vi "Language Editor.vi"(8 "error in (no error)":errorcluster, 11 "Top Level VI":refnum<vi>) -> (0 "error out":errorcluster)   [LabVIEW 2019, in "Language Editor.lvlib"]
doc: "- - -\nCopyright (c) 2026, Merecs Engineering GmbH"
uses:
  Language Editor.lvlib
  type defs/Enum Class Name.ctl
  Language Selection/TypeDefs/Cluster Language Configuration.ctl
  Language Selection/community/Cluster Settings Data.ctl
  Language Selection/TypeDefs/Cluster Language.ctl
  Language Selection/TypeDefs/Cluster PropertyTranslation.ctl
  Language Selection/TypeDefs/Enum Property Type.ctl
  type defs/Cluster VI controls.ctl
  type defs/Cluster Translations.ctl
  <vilib>/Utility/miscctls.llb/LVPointTypeDef.ctl
  <vilib>/Utility/miscctls.llb/LVRowAndColumnUnsignedTypeDef.ctl
  <vilib>/Utility/miscctls.llb/LVBoundsTypeDef.ctl
  <vilib>/Utility/miscctls.llb/LVMapReplaceAction.ctl
  70223300-0df1-46fa-af21-f54e94af5b86.vi
  <vilib>/addons/Tools/Unicode/_subVIs/Convert UTF-16LE to ASCII (Scalar).vi
  Language Selection/Language Selection.lvlib
  <vilib>/addons/Tools/Unicode/UI Unicode Tools.lvlib
  <vilib>/Utility/LVLibp/NI_PackedLibraryUtility.lvlib
panel:
  in  "Import":bool
  in  "Export to txt":bool
  in  "App File Path":path=path "C:/Projects/Base/Modules/Language Toolkit" caption="Application Base Folder Path"
  in  "Save As":bool
  in  "Language Config Path":path=path "C:/Projects/Base/Modules/Language Toolkit/data/Language Translation_default.json"
  in  "Save Settings":bool
  in  "Init":bool
  in  "Exit":bool
  in  "Tab Control":T1(tab)
  in  "StartLang":string(combo) caption="Startup Language"
  in  "DefLang":string(combo) caption="Default Language"
  in  "Delete":bool
  in  "AddLanguage":bool
  in  "Languages":i32(listbox) caption="Languages to translate"
  in  "Search":string
  in  "AllLanguages":i32(listbox)=-1 caption="List of languages"
  in  "VI.DelAllFilter":bool
  in  "Button.GoToTranslation":bool
  in  "Add VI":bool caption="Last"
  in  "Sort VIs":bool
  in  "Delete VI":bool caption="First"
  in  "Button.AddToFPTranslation":bool
  in  "ControlsFilter":T2={"VI.Filter.Label"="num", "VI.Filter.Class"="", "No Error Cluster"=TRUE, "NonTranslated"=TRUE, "OnlyVisibleArea"=TRUE} caption="Controls Filter"
  in  "Controls":i32[](listbox)
  in  "VIs":i32(listbox) caption="VIs to translate"
  out "IsCtrlVisible":bool
  in  "Search Label":string
  in  "DelFilter":bool
  out "Warning":string
  in  "FPT.TextUnicode":string caption="Translation"
  in  "CTRL Index":i32 caption="Control Index" min=0 max=26 step=1
  in  "ListOfControls":i32(listbox) caption="List Of Controls"
  out "Caption Unvisible":bool
  in  "FP Translation Comment":string caption="Comment"
  out "IsCtrlUsed":bool
  out "Class Name":T3=enum."ListBox"
  in  "Button.NextUnusedCtrls":bool
  in  "VIs with Ctrl":i32(listbox) caption="List of UIs with control:"
  in  "Button.ZoomToCtrl":bool
  out "2D Picture":picture
  in  "Tree":string(tree)="TipStrip"
  in  "DelCtrlToTranslate":bool caption="First"
  in  "AddCtrlToTranslate":bool caption="Last"
  in  "Label":string="L.Listbox"
  in  "FPT.TextANSI":string caption="Translation"
  out "IsCtrlInUIArea":bool
  in  "TT.TextUnicode":string caption="Translation"
  in  "TextTranslation":i32(listbox)
  in  "TT.TextANSI":string caption="Translation"
  in  "ListOfTextTranslations":i32(listbox)=-1
  in  "DeleteText":bool caption="First"
  in  "AddTextToTranslate":bool caption="Last"
  in  "TextName":string="L.Listbox" caption="Name"
  in  "Search text":string
  # "Select Language"
  # "Language Preferences"
  # "Double Click to Show VI Frontpanel"
  # "Connector Pane"
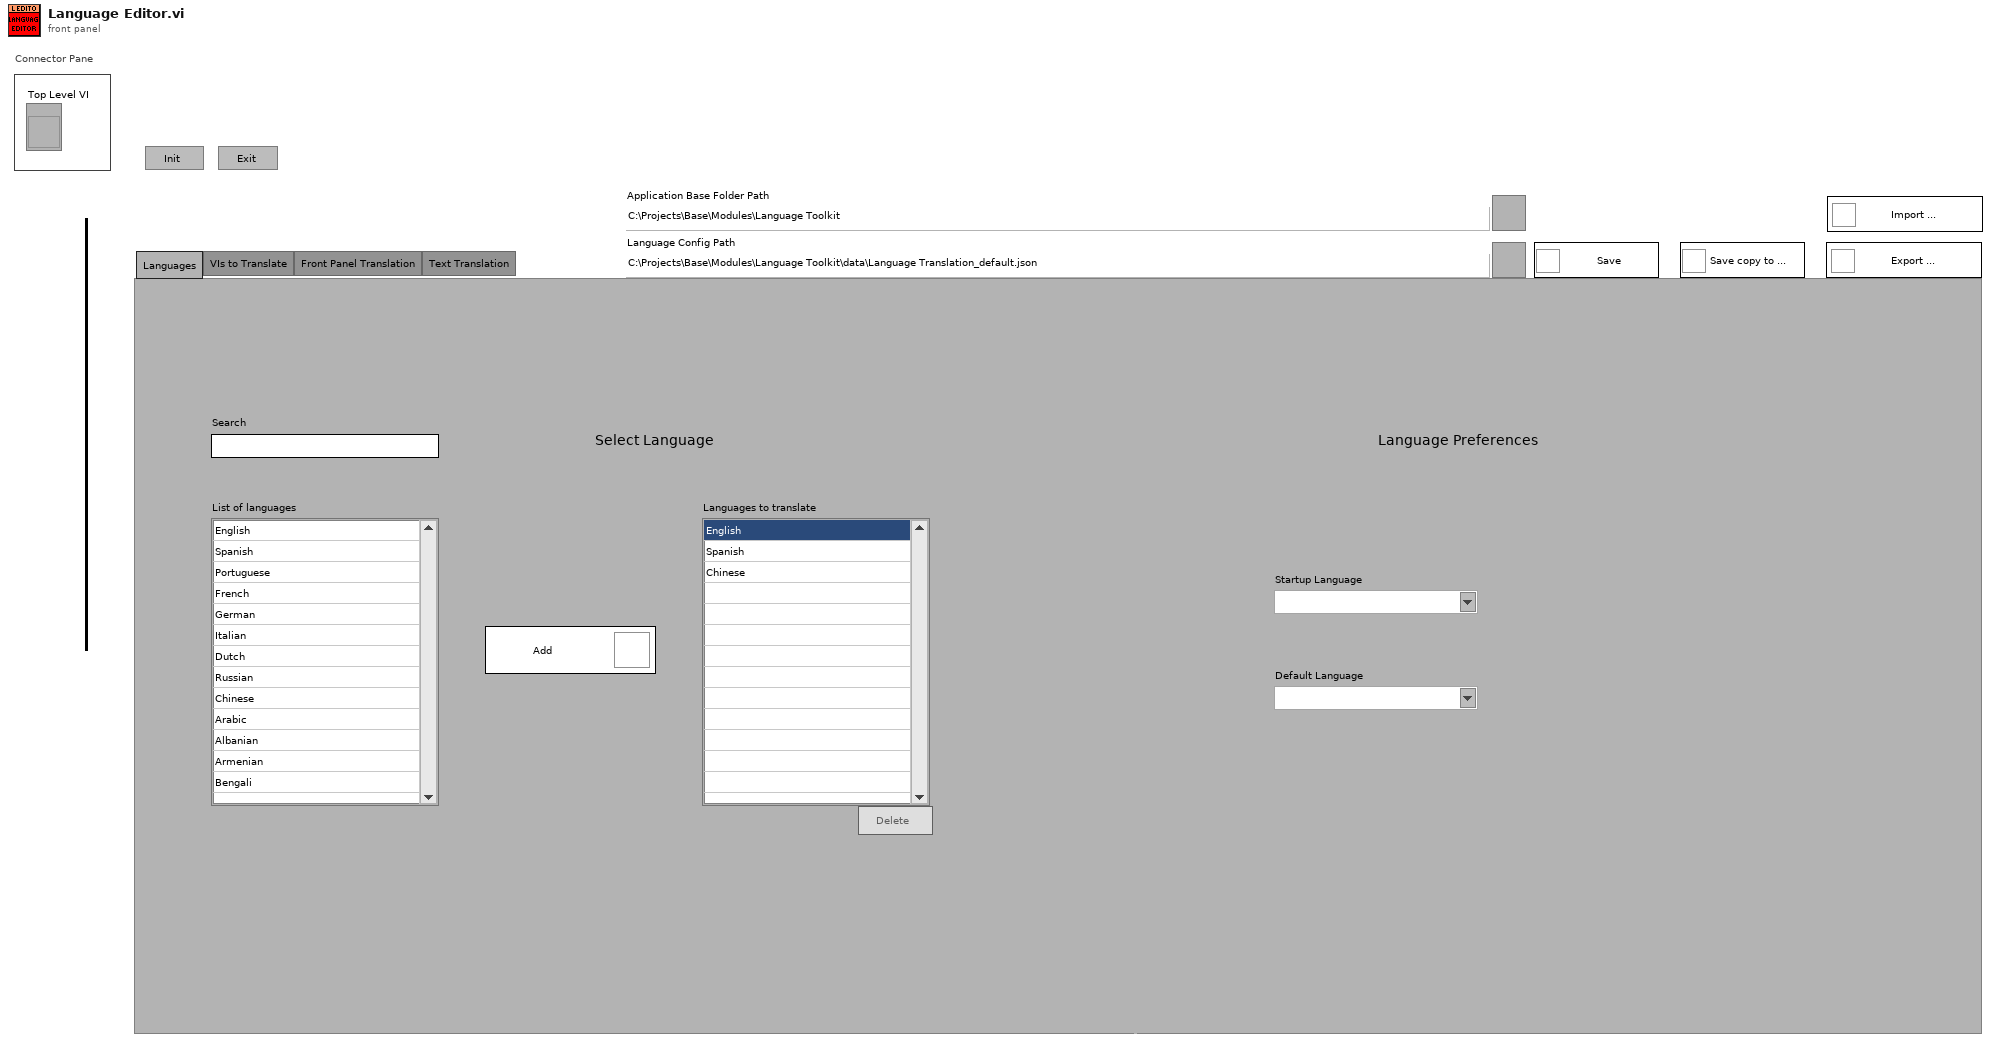
[diagram p1: front panel]
types:
  T1 = enum32{"Languages", "VIs to Translate", "Front Panel Translation", "Text Translation"}
  T2 = cluster{"VI.Filter.Label":string, "VI.Filter.Class":string, "No Error Cluster":bool, "NonTranslated":bool, "OnlyVisibleArea":bool}
  T3 = typedef "Language Editor.lvlib/Enum Class Name.ctl" = enum16{"Default Control", "Boolean", "ListBox", "Table", "Graph", "Array", "Ring", "String", "TabControl", "ComboBox", "TreeControl"}
  T4 = enum8{"Enabled", "Disabled", "Disabled and Grayed Out"}
  T5 = enum32{"Invalid", "Standard", "Closed", "Hidden", "Minimized", "Maximized"}
  T6 = enum32{"invalid app kind", "Development System", "Run Time System", "Student Edition", "Embedded LabVIEW", "Evaluation", "Custom"}
  T7 = typedef "Language Selection.lvlib/Cluster Language.ctl" = cluster{"Label":string, "Comment":string, "Property":T8[]}
  T8 = typedef "Language Selection.lvlib/Cluster PropertyTranslation.ctl" = cluster{"Type":T9, "Translation ANSI":string[], "Translation Unicode":string[]}
  T9 = typedef "Language Selection.lvlib/Enum Property Type.ctl" = enum16{"NA", "Caption", "String Value", "Boolean Text", "Ring Strings", "1D Array Elements", "2D Array Elements", "(MC)Listbox Header", "(MC)Listbox Items", "Tab Pages Names", "X & Y GraphChart", "Plot Names", "Table Headers", "Table Items", "TipStrip", "Combobox Strings", "Cursor Name", "Tree Col Headers"}
  T10 = typedef "LVPointTypeDef.ctl" = cluster{"Horizontal":i16, "Vertical":i16}
  T11 = typedef "LVRowAndColumnUnsignedTypeDef.ctl" = cluster{"Row":u32, "Column":u32}
  T12 = typedef "LVBoundsTypeDef.ctl" = cluster{"Width":u32, "Height":u32}
  T13 = typedef "LVMapReplaceAction.ctl" = enum32{"Modify Entry only if found", "Add or Modify Entry", "Delete Entry"}
  T14 = typedef "Language Editor.lvlib/Cluster Translations.ctl" = cluster{"Tags":string, "Comment":string, "Properties":T8[]}
  T15 = typedef "Language Selection.lvlib/Cluster Language Configuration.ctl" = cluster{"Data":T16, "Supported Languages":cluster{"ANSI":string[], "Unicode":string[]}, "VIs":path[], "FP Translations":T7[], "Text Translations":T7[]}
  T16 = typedef "Language Selection.lvlib/Cluster Settings Data.ctl" = cluster{"Startup Language":string, "Default Language":string, "Languages":cluster{"ANSI":string[], "Unicode":string[]}}
  T17 = typedef "Language Editor.lvlib/Cluster VI controls.ctl" = cluster{"Label":string, "Class Name":string, "Type":string, "Tags":string, "refVI":refnum<vi>, "refCtl":refnum<vi>, "PageOfTab":string, "refPane":refnum<vi>}
  T18 = cluster{"Core":cluster{"Current VI Reference":refnum<vi>, "Close Panel on Exit?":bool}, "LT":T15, "CTRLs":map{path, T17[]}, "Controls":cluster{"Item Names":string[][], "Item Symbols":i32[]}, "Selected CTRLs":T17[], "OldVal.ListOfVIs":string, "ZoomOutFactor":dbl, "FP.Tr":map{string, T14}, "T.Tr":map{string, T14}, "Origin":T10}
  T19 = cluster{"Current VI Reference":refnum<vi>, "Close Panel on Exit?":bool}
  T20 = cluster{"Item Names":string[][], "Item Symbols":i32[]}
  T21 = cluster{"Left Cell String":string, "Child Text":string[], "Child Tag":string, "Item Indent":i32, "Child Only?":bool, "Glyph Index":i32}[]
  T22 = cluster{"left":i16, "top":i16, "right":i16, "bottom":i16}
  T23 = enum16{"open", "replace", "create", "open or create", "replace or create", "replace or create with confirmation"}
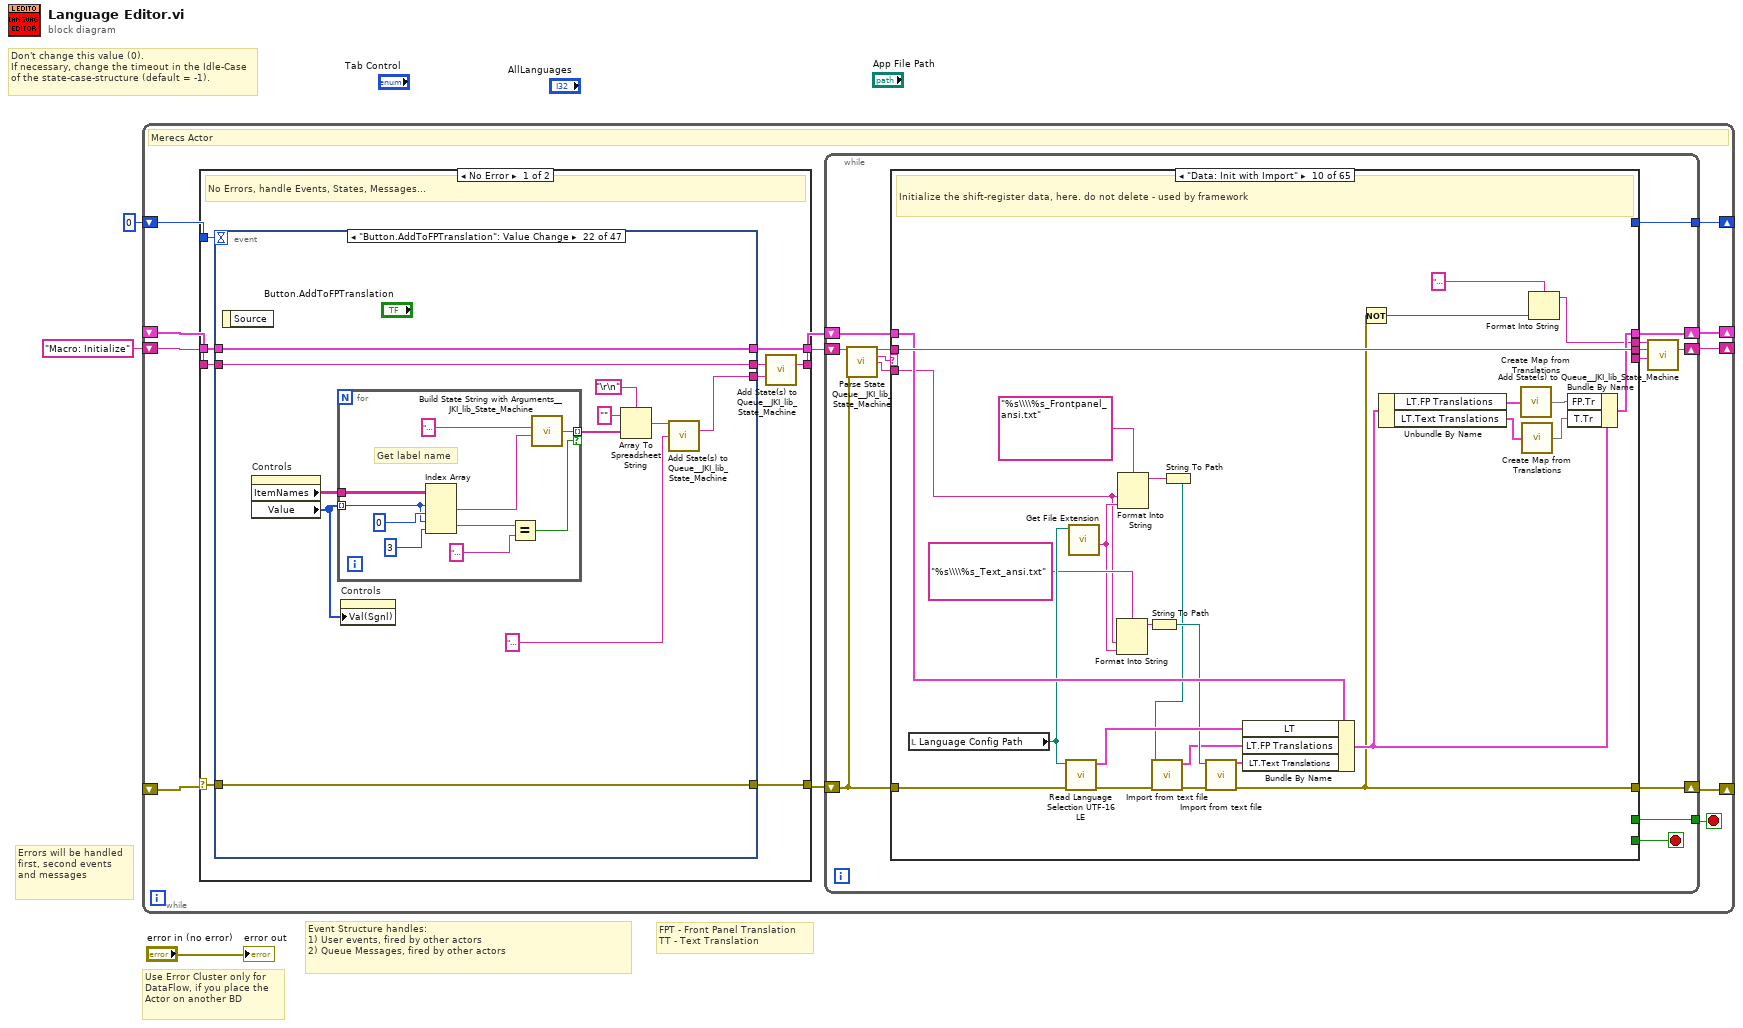
[diagram p0: block diagram]
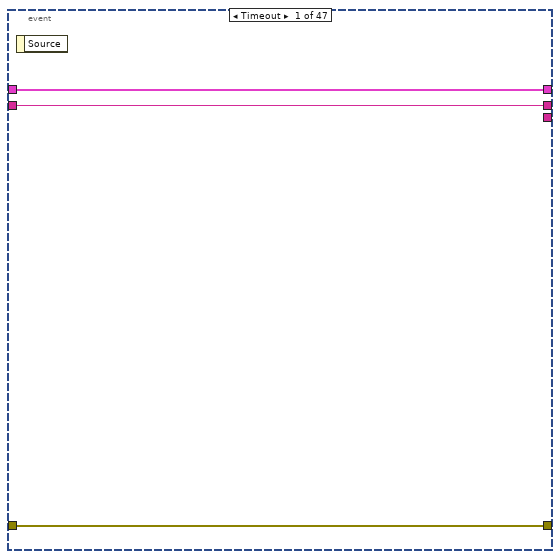
[diagram p2: hidden frame]
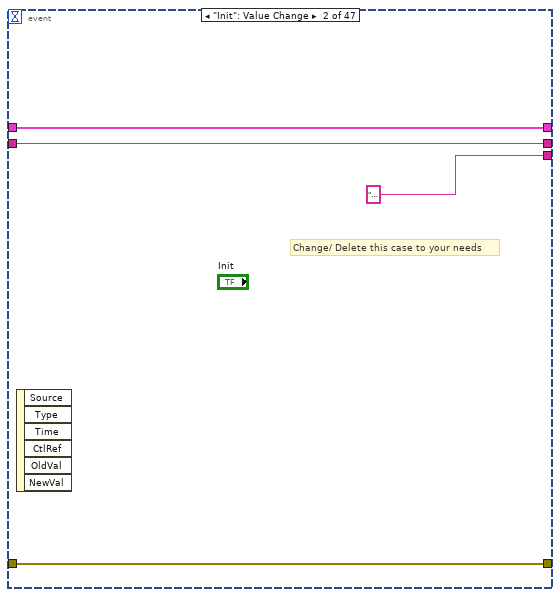
[diagram p3: hidden frame]
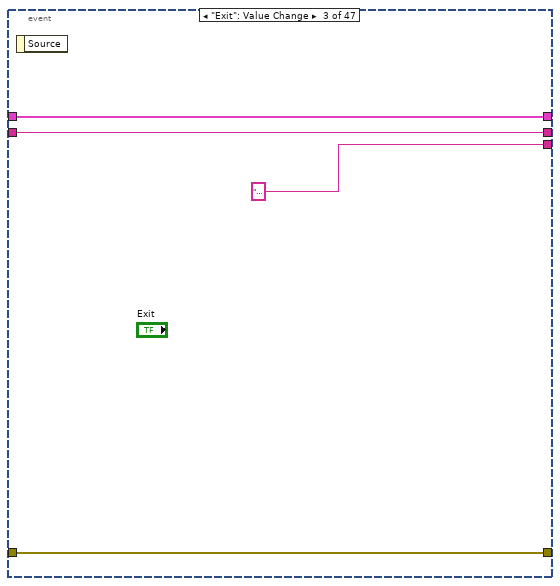
[diagram p4: hidden frame]
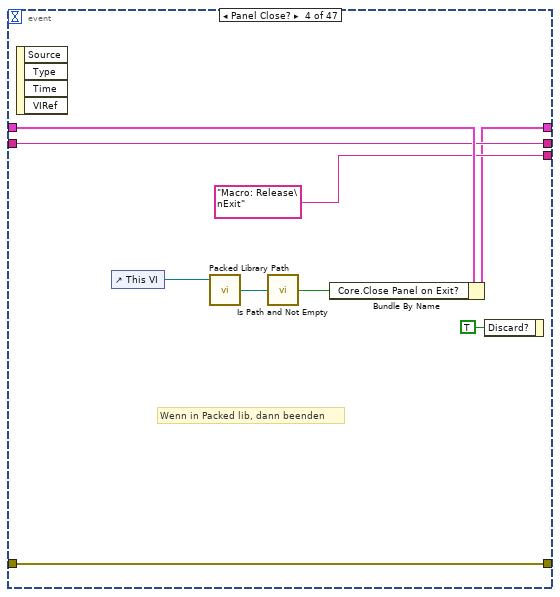
[diagram p5: hidden frame]
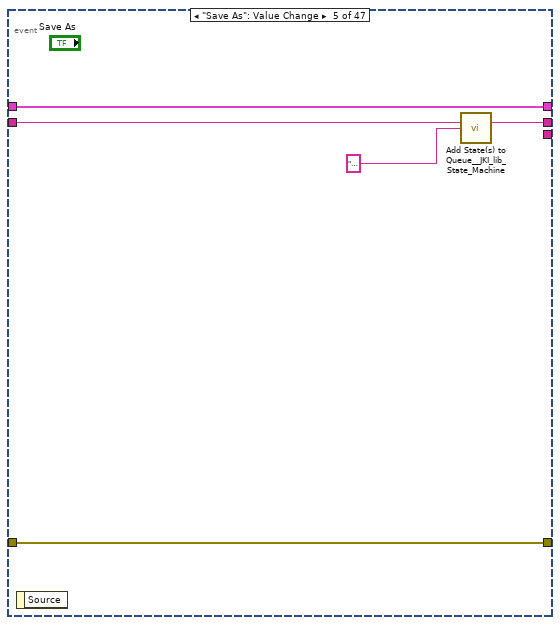
[diagram p6: hidden frame]
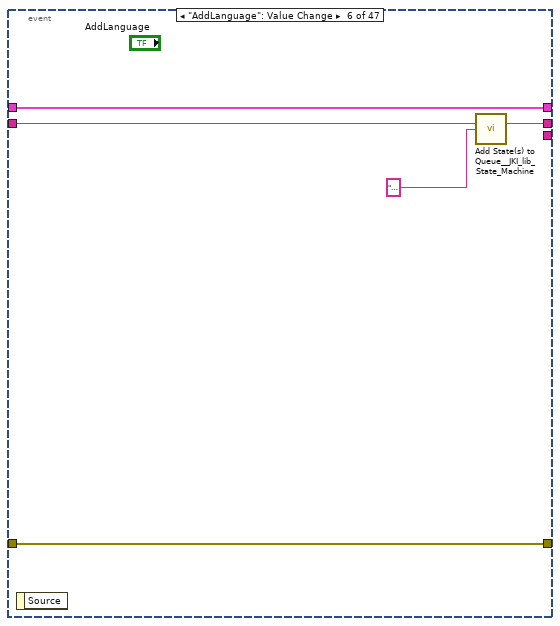
[diagram p7: hidden frame]
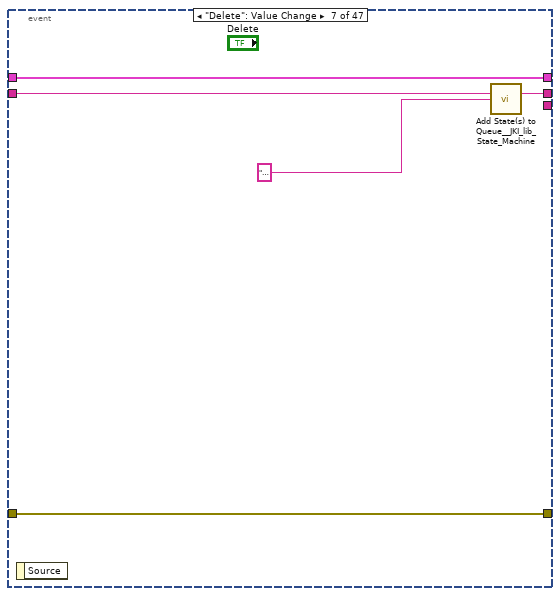
[diagram p8: hidden frame]
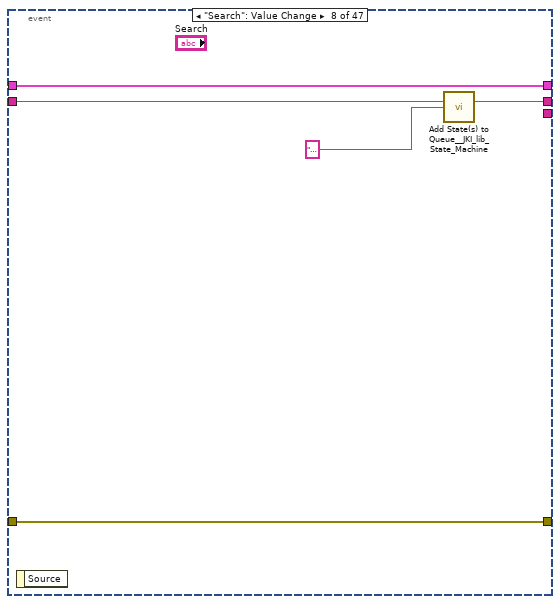
[diagram p9: hidden frame]
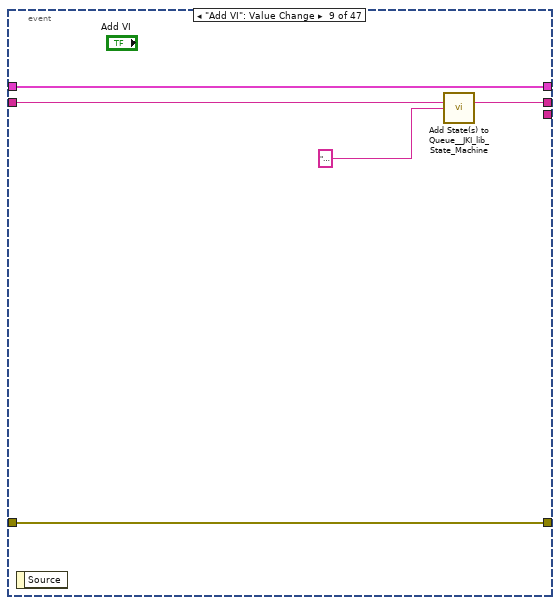
[diagram p10: hidden frame]
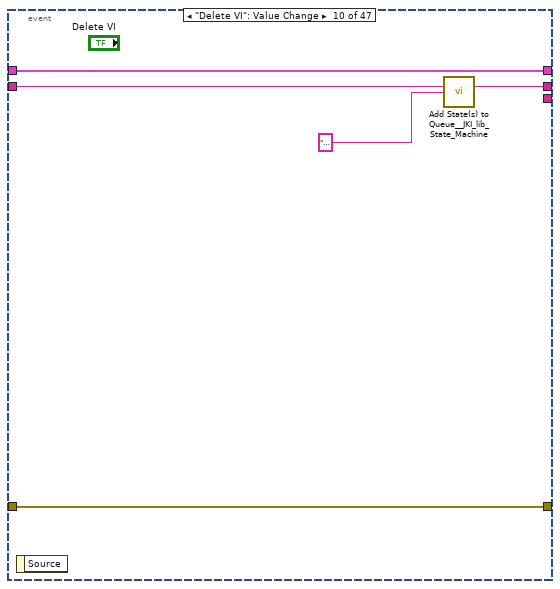
[diagram p11: hidden frame]
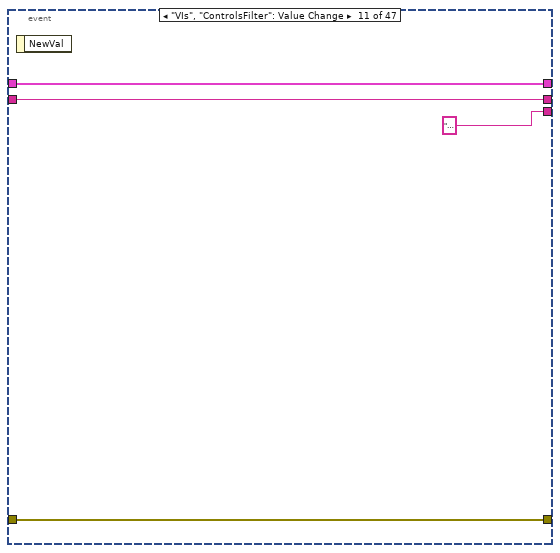
[diagram p12: hidden frame]
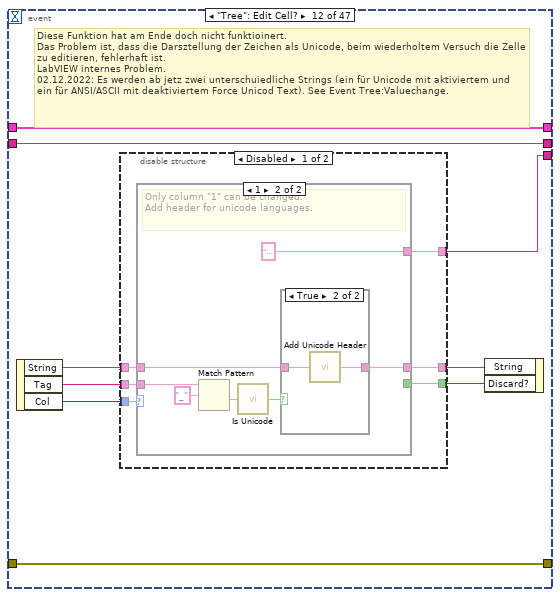
[diagram p13: hidden frame]
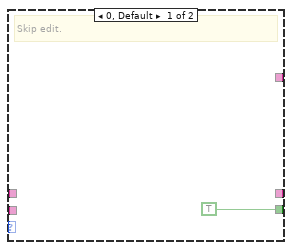
[diagram p14: hidden frame]
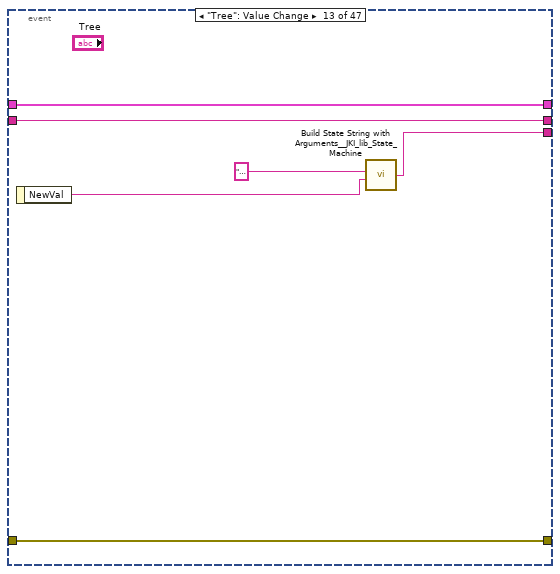
[diagram p17: hidden frame]
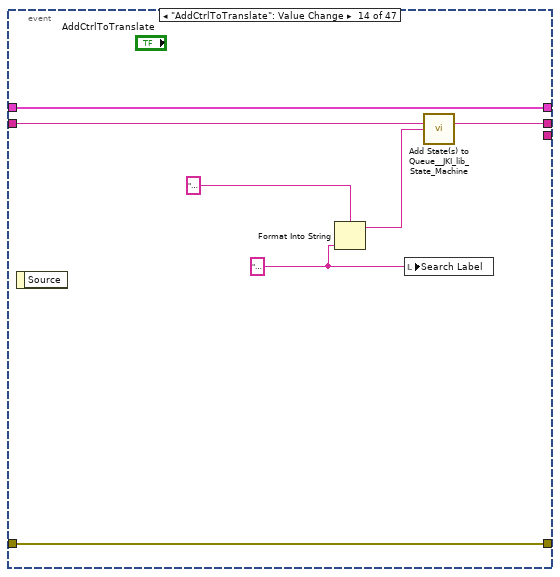
[diagram p18: hidden frame]
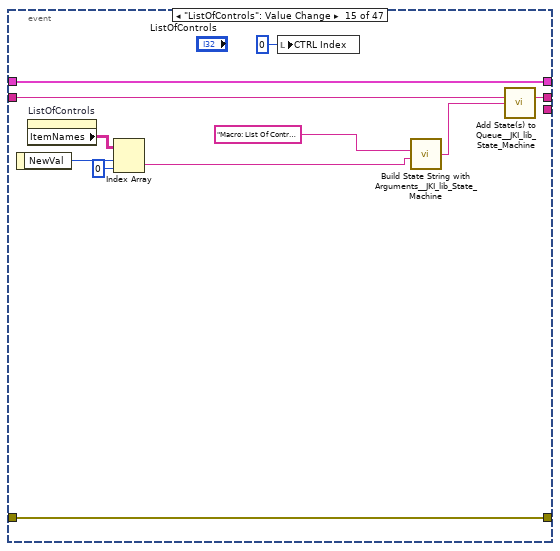
[diagram p19: hidden frame]
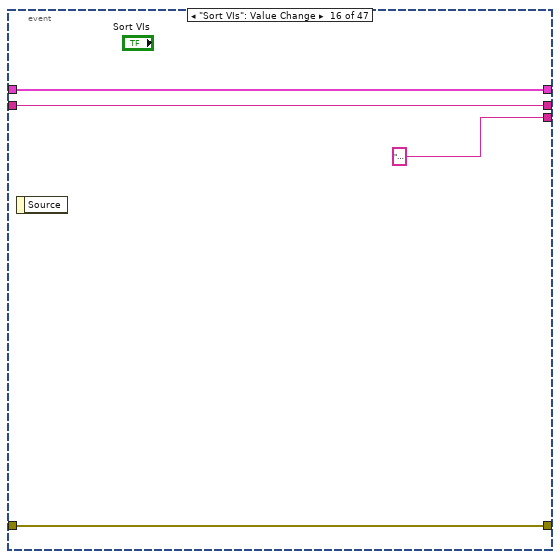
[diagram p20: hidden frame]
diagram:
  # "FPT - Front Panel Translation\nTT - Text Translation"
  # "Errors will be handled first, second events and messages"
  # "Use Error Cluster only for DataFlow, if you place the Actor on another BD"
  # "Event Structure handles:\n1) User events, fired by other actors\n2) Queue Messages, fired by other actors"
  # "Don't change this value (0).\nIf necessary, change the timeout in the Idle-Case of the state-case-structure (default = -1)."
  n1 = while {
    shift-right: [w15] -> _
    shift-left: _ -> [w13]
    shift-right: [w5] -> _
    shift-left: 0 -> [w8]
    shift-right: [w7] -> _
    shift-left: "Macro: Initialize" ("States Out") -> [w6]
    shift-right: [w14] -> _
    shift-left: _ -> [w4]
    stop <- w10 stop-if-true
    # "Merecs Actor"
    n2 = case shown="No Error" w4 {
      selector: w4 -> [w19 w362]
      tunnel: w13 -> [w24 w364]
      tunnel: [w23 w364] -> w12
      tunnel: [w18 w363] -> w11
      tunnel: [w22 w362] -> w9
      tunnel: w8 -> [w21 _]
      tunnel: w6 -> [w20 w363]
      frame No Error {
        # "No Errors, handle Events, States, Messages..."
        n3 = event shown="[21] \"Button.AddToFPTranslation\": Value Change" {
          selector: _ -> [_ _ _ _ _ _ _ _ _ _ _ _ _ _ _ _ _ _ _ _ _ _ _ _ _ _ _ _ _ _ _ _ _ _ _ _ _ _ _ _ _ _ _ _ _ _ _]
          dyn-events: _ -> [_ _ _ _ _ _ _ _ _ _ _ _ _ _ _ _ _ _ _ _ _ _ _ _ _ _ _ _ _ _ _ _ _ _ _ _ _ _ _ _ _ _ _ _ _ _ _]
          timeout: w21 -> [_ _ _ _ _ _ _ _ _ _ _ _ _ _ _ _ _ _ _ _ _ _ _ _ _ _ _ _ _ _ _ _ _ _ _ _ _ _ _ _ _ _ _ _ _ _ _]
          tunnel: w24 -> [w27 w31 w34 w43 w49 w54 w59 w64 w69 w74 w78 w87 w110 w117 w128 w132 w140 w145 w150 w155 w162 w173 w189 w197 w201 w205 w214 w221 w230 w234 w238 w242 w246 w250 w254 w266 w276 w283 w287 w294 w324 w328 w332 w336 w344 w349 w357]
          tunnel: [w27 w31 w34 w37 w49 w54 w59 w64 w69 w74 w78 w87 w110 w117 w128 w132 w140 w142 w147 w155 w162 w173 w189 w197 w201 w205 w209 w221 w230 w234 w238 w242 w246 w250 w254 w266 w276 w283 w287 w294 w324 w328 w332 w336 w344 w349 w357] -> w23
          tunnel: [w25 w28 w32 w41 w46 w50 w56 w62 w67 w72 w77 w86 w109 w115 w125 w131 w139 w144 w149 w154 w161 w172 w188 w196 w200 w204 w211 w220 w229 w233 w237 w241 w245 w249 w253 w265 w275 w282 w286 w293 w323 w327 w331 w335 w343 w348 w356] -> w16
          tunnel: w19 -> [w26 w30 w35 w44 w48 w53 w58 w63 w68 w73 w76 w85 w108 w116 w127 w130 w138 w143 w148 w153 w160 w171 w187 w195 w199 w203 w213 w219 w228 w232 w236 w240 w244 w248 w252 w264 w274 w281 w285 w292 w322 w326 w330 w334 w342 w347 w351]
          tunnel: [w26 w30 w35 w44 w48 w53 w58 w63 w68 w73 w76 w85 w108 w116 w127 w130 w138 w143 w148 w153 w160 w171 w187 w195 w199 w203 w213 w219 w228 w232 w236 w240 w244 w248 w252 w264 w274 w281 w285 w292 w322 w326 w330 w334 w342 w347 w350] -> w22
          tunnel: w20 -> [w25 w28 w32 w41 w47 w51 w57 w61 w66 w71 w77 w86 w109 w114 w126 w131 w139 w144 w149 w154 w161 w172 w188 w196 w200 w204 w210 w220 w229 w233 w237 w241 w245 w249 w253 w265 w275 w282 w286 w293 w323 w327 w331 w335 w343 w348 w356]
          tunnel: [_ "Macro: Initialize" ("State(s) at Back (\"\")") "Macro: Release\nExit" ("State(s) at Back (\"\")") "Macro: Release\nExit" ("State(s) at Back (\"\")") _ _ _ _ _ _ "UI: VIs Update Controls" ("State") w79 w105 _ _ "VIs: Sort\nUI: VIs Update" ("State with Arguments") w134 _ _ _ "UI: VIs Update Controls" ("State with Arguments") w169 "FP Translation: Edit Properties\nUI: FP Translation Filter ListOfControls" ("State with Arguments") "FP Translation: Edit Properties\nUI: FP Translation Filter ListOfControls" ("State with Arguments") "FP Translation: Delete Control" ("State") "FP Translation: Look for Next unused CTRL" _ w216 w222 "Data: FP Translation Edit Comment" ("State") "UI: FP Translation Filter ListOfControls" ("State") "Text Translation: Show Translation\nText Translation: Value Change" ("State") "Text Translation: Add Text >> New Text" ("State(s) at Back (\"\")") "Text Translation: Delete Text" ("State(s) at Back (\"\")") "Text Translation: Value Change" ("f") "Text Translation: Edit Properties" ("State(s) at Back (\"\")") "Text Translation: Edit Properties" ("State(s) at Back (\"\")") w278 "Data: Update Config\nData: Save" ("State with Arguments") _ w314 "VIs: Show Frontpanel" ("State with Arguments") "Text Translation: Filter" ("State with Arguments") _ w338 "General: Export to txt" ("f") w355] -> w17
          event Timeout {
            n4 = event-data() -> ()  [unwired: 1 in, 1 out]
          }
          event "Init": Value Change {
            # "Change/ Delete this case to your needs"
            n5 = event-data() -> ()  [unwired: 1 in, 6 out]
          }
          event "Exit": Value Change {
            n6 = event-data() -> ()  [unwired: 1 in, 1 out]
          }
          event Panel Close? {
            # "Wenn in Packed lib, dann beenden"
            n7 = event-data() -> ()  [unwired: 1 in, 4 out]
            n8 = control-ref of="This VI"() -> (w39:refnum<vi>)
            n9 = call <vilib>:"Packed Library Path.vi"("vi reference"=w39) -> ("packed library path"=w38:path)  [unwired: 2 in, 2 out]
            n10 = call <vilib>:"Is Path and Not Empty.vi"("path"=w38) -> ("Is Path and Not Empty?"=w36:bool)  [unwired: 4 in]
            n11 = Bundle By Name(cluster=w43, "Core.Close Panel on Exit?"=w36) -> (w37:T18)
            n12 = event-data("Discard?"=TRUE) -> ()  [unwired: 1 in, 1 out]
          }
          event "Save As": Value Change {
            n13 = event-data() -> ()  [unwired: 1 in, 1 out]
            n14 = call <vilib>:"Add State(s) to Queue__JKI_lib_State_Machine.vi"("State(s) in (\"\")"=w47, "State(s) at Back (\"\")"="General: File Save As" ("State(s) at Back (\"\")")) -> ("States Out"=w46:string)  [unwired: 13 in]
          }
          event "AddLanguage": Value Change {
            n15 = event-data() -> ()  [unwired: 1 in, 1 out]
            n16 = call <vilib>:"Add State(s) to Queue__JKI_lib_State_Machine.vi"("State(s) in (\"\")"=w51, "State(s) at Back (\"\")"="Languages: Add\nUI: Languages" ("State(s) at Back (\"\")")) -> ("States Out"=w50:string)  [unwired: 13 in]
          }
          event "Delete": Value Change {
            n17 = event-data() -> ()  [unwired: 1 in, 1 out]
            n18 = call <vilib>:"Add State(s) to Queue__JKI_lib_State_Machine.vi"("State(s) in (\"\")"=w57, "State(s) at Back (\"\")"="Languages: Delete\nUI: Languages" ("State(s) at Back (\"\")")) -> ("States Out"=w56:string)  [unwired: 13 in]
          }
          event "Search": Value Change {
            n19 = event-data() -> ()  [unwired: 1 in, 1 out]
            n20 = call <vilib>:"Add State(s) to Queue__JKI_lib_State_Machine.vi"("State(s) in (\"\")"=w61, "State(s) at Back (\"\")"="Languages: Search" ("State(s) at Back (\"\")")) -> ("States Out"=w62:string)  [unwired: 13 in]
          }
          event "Add VI": Value Change {
            n21 = event-data() -> ()  [unwired: 1 in, 1 out]
            n22 = call <vilib>:"Add State(s) to Queue__JKI_lib_State_Machine.vi"("State(s) in (\"\")"=w66, "State(s) at Back (\"\")"=" VIs: Add VI\nUI: VIs Update" ("State(s) at Back (\"\")")) -> ("States Out"=w67:string)  [unwired: 13 in]
          }
          event "Delete VI": Value Change {
            n23 = event-data() -> ()  [unwired: 1 in, 1 out]
            n24 = call <vilib>:"Add State(s) to Queue__JKI_lib_State_Machine.vi"("State(s) in (\"\")"=w71, "State(s) at Back (\"\")"="VIs: Delete VI\nUI: VIs Update" ("State(s) at Back (\"\")")) -> ("States Out"=w72:string)  [unwired: 13 in]
          }
          event "VIs", "ControlsFilter": Value Change {
            n25 = event-data() -> ()  [unwired: 1 in, 1 out]
          }
          event "Tree": Edit Cell? {
            # "Diese Funktion hat am Ende doch nicht funktioinert.\nDas Problem ist, dass die Darsztellung der Zeichen als Unicode, beim wiederholtem Versuch die Zelle zu editieren, fehlerhaft ist.\nLabVIEW internes Problem.\n02.12.2022: Es werden ab jetz zwei unterschuiedliche Strings (ein für Unicode mit aktiviertem und ein für ANSI/ASCII mit deaktiviertem Force Unicod Text). See Event Tree:Valuechange."
            n26 = event-data() -> ("String"=w81:string, "Tag"=w82:string, "Col"=w84:i32)  [unwired: 1 in]
            n27 = disable-structure shown="Disabled" {
              disable-tunnel: w84 -> [w93 _]
              disable-tunnel: [w92 _] -> w83
              disable-tunnel: w82 -> [w91 _]
              disable-tunnel: w81 -> [w90 _]
              disable-tunnel: [w89 _] -> w80
              disable-tunnel: [w88 _] -> w79
              frame Disabled {
                n28 = case shown="1" w93 {
                  tunnel: [TRUE _] -> w92
                  tunnel: w91 -> [_ w98]
                  tunnel: w90 -> [_ w97]
                  tunnel: [_ w96] -> w89
                  tunnel: [_ "FP Translation: Edit Properties" ("State with Arguments")] -> w88
                  frame 0, Default {
                    # "Skip edit."
                  }
                  frame 1 {
                    # "Only column \"1\" can be changed.\nAdd header for unicode languages."
                    n29 = Match Pattern(string=w98, regular expression="_") -> (after substring=w100:string)  [unwired: 1 in, 3 out]
                    n30 = call "Is Unicode.vi"("Language"=w100) -> ("Is Unicode"=w99:bool)
                    n31 = case shown="True" w99 {
                      tunnel: [w102 w103] -> w96
                      tunnel: w97 -> [w102 w104]
                      frame False {
                      }
                      frame True {
                        n32 = call "Add Unicode Header.vi"("Text"=w104) -> ("Text with header"=w103:string)
                      }
                    }
                  }
                }
              }
              frame Enabled {
              }
            }
            n33 = event-data("String"=w80, "Discard?"=w83) -> ()  [unwired: 1 in, 1 out]
          }
          event "Tree": Value Change {
            n34 = event-data() -> ("NewVal"=w106:string)  [unwired: 1 in]
            n35 = call <vilib>:"Build State String with Arguments__JKI_lib_State_Machine.vi"("Arguments (\"\")"=w106, "State"="UI: FP Translation Update Text Translations") -> ("State with Arguments"=w105:string)  [unwired: 4 in]
          }
          event "AddCtrlToTranslate": Value Change {
            w113 = "New Label" ("Search Label")
            n36 = event-data() -> ()  [unwired: 1 in, 1 out]
            n37 = Format Into String(format string="FP Translation: Add Control >> %s\nUI: FP Translation Filter ListOfControls" ("State(s) at Back (\"\")"), w113) -> (resulting string=w111:string)  [unwired: 2 in, 1 out]
            n38 = local write "Search Label"(w113) -> ()
            n39 = call <vilib>:"Add State(s) to Queue__JKI_lib_State_Machine.vi"("State(s) in (\"\")"=w114, "State(s) at Back (\"\")"=w111) -> ("States Out"=w115:string)  [unwired: 13 in]
          }
          event "ListOfControls": Value Change {
            n40 = event-data() -> ("NewVal"=w123:i32)  [unwired: 1 in]
            n41 = property on="ListOfControls" class="MCListbox (strict)"() -> ("ItemNames"=w121:string[][])  [unwired: 2 in, 2 out]
            n42 = Index Array(array=w121, index (row)=w123, index (col)=0 ("disabled index (col)")) -> (element=w119:string)
            n43 = local write "CTRL Index"(0 ("CTRL Index")) -> ()
            n44 = call <vilib>:"Build State String with Arguments__JKI_lib_State_Machine.vi"("Arguments (\"\")"=w119, "State"="Macro: List Of Controls Value Change") -> ("State with Arguments"=w120:string)  [unwired: 4 in]
            n45 = call <vilib>:"Add State(s) to Queue__JKI_lib_State_Machine.vi"("State(s) in (\"\")"=w126, "State(s) at Back (\"\")"=w120) -> ("States Out"=w125:string)  [unwired: 13 in]
          }
          event "Sort VIs": Value Change {
            n46 = event-data() -> ()  [unwired: 1 in, 1 out]
          }
          event "Label": Value Change {
            n47 = event-data() -> ("NewVal"=w133:string)  [unwired: 1 in]
            n48 = local write "Search Label"(w133) -> ()
            n49 = call <vilib>:"Build State String with Arguments__JKI_lib_State_Machine.vi"("Arguments (\"\")"=w133, "State"="FP Translation: Rename Control") -> ("State with Arguments"=w135:string)  [unwired: 4 in]
            n50 = call <vilib>:"Add State(s) to Queue__JKI_lib_State_Machine.vi"("State(s) in Front (\"\")"=w135, "State(s) in (\"\")"="UI: FP Translation Filter ListOfControls" ("State(s) in (\"\")")) -> ("States Out"=w134:string)  [unwired: 13 in]
          }
          event "StartLang": Value Change {
            n51 = event-data() -> ("NewVal"=w141:string)  [unwired: 1 in]
            n52 = Bundle By Name(cluster=w145, "LT.Data.Startup Language"=w141) -> (w142:T18)
          }
          event "DefLang": Value Change {
            n53 = event-data() -> ("NewVal"=w146:string)  [unwired: 1 in]
            n54 = Bundle By Name(cluster=w150, "LT.Data.Default Language"=w146) -> (w147:T18)
          }
          event "Languages": Value Change {
            n55 = event-data() -> ("NewVal"=w152:i32)  [unwired: 1 in]
            n56 = case shown="-1" w152 {
              tunnel: [T4."Disabled and Grayed Out" ("Disabled") T4."Enabled" ("Disabled")] -> w151
              frame -1 {
              }
              frame Default {
              }
            }
            n57 = property on="Delete" class="Bool"("DisabledEnum"=w151) -> ()  [unwired: 2 in, 2 out]
          }
          event "VI.DelAllFilter": Value Change {
            n58 = event-data() -> ()  [unwired: 1 in, 1 out]
            n59 = local write "ControlsFilter"(T2 {"VI.Filter.Label"="", "VI.Filter.Class"="", "No Error Cluster"=FALSE, "NonTranslated"=FALSE, "OnlyVisibleArea"=FALSE} ("ControlsFilter")) -> ()
          }
          event "Button.AddToFPTranslation": Value Change {
            n60 = event-data() -> ()  [unwired: 1 in, 1 out]
            n61 = property on="Controls" class="MCListbox (strict)"() -> ("ItemNames"=w170:string[][], "Value"=w167:i32[])  [unwired: 2 in, 2 out]
            n62 = for {
              tunnel: w170 -> [w182]
              tunnel: [w179] -> w166 mode=indexing if=w177
              tunnel: w167 -> [w176] mode=indexing
              # "Get label name"
              n63 = Index Array(array=w182, index (row) #1=w176, index (col) #1=0 ("disabled index (col)"), index (row) #2=w176, index (col) #2=3 ("disabled index (col)")) -> (element #1=w180:string, element #2=w174:string)
              n64 = Equal?(x=w174, y="Not Added") -> (x = y?=w177:bool)
              n65 = call <vilib>:"Build State String with Arguments__JKI_lib_State_Machine.vi"("Arguments (\"\")"=w180, "State"="FP Translation: Add Control") -> ("State with Arguments"=w179:string)  [unwired: 4 in]
            }
            n66 = property on="Controls" class="MCListbox (strict)"("Val(Sgnl)"=w167) -> ()  [unwired: 2 in, 2 out]
            n67 = Array To Spreadsheet String(delimiter (Tab)="\r\n", array=w166, 3:"" ("format string")) -> (spreadsheet string=w165:string)
            n68 = call <vilib>:"Add State(s) to Queue__JKI_lib_State_Machine.vi"("State(s) in Front (\"\")"=w165, "State(s) at Back (\"\")"="UI: VIs Update Controls" ("State(s) at Back (\"\")")) -> ("States Out"=w169:string)  [unwired: 13 in]
          }
          event "FPT.TextUnicode": Value Change {
            n69 = event-data() -> ("NewVal"=w185:string)  [unwired: 1 in]
            n70 = call "Add Unicode Header.vi"("Text"=w185) -> ("Text with header"=w186:string)  [unwired: 1 in, 1 out]
            n71 = property on="Tree" class="Tree (strict)"("Cell String"=w186) -> ()  [unwired: 2 in, 2 out]
          }
          event "FPT.TextANSI": Value Change {
            # "Delete NULL bytes from string.\nLabVIEW bug: Some times inserts LabVIEW NULL bytes by paste with Ctr-V."
            n72 = event-data() -> ("NewVal"=w191:string)  [unwired: 1 in]
            n73 = Search and Replace String(replace all?=TRUE ("replace all? (F)"), input string=w191, search string="\u0000") -> (result string=w190:string)  [unwired: 5 in, 3 out]
            n74 = property on="Tree" class="Tree (strict)"("Cell String"=w190) -> ()  [unwired: 2 in, 2 out]
            n75 = local write "FPT.TextANSI"(w190) -> ()
          }
          event "DelCtrlToTranslate": Value Change {
            n76 = event-data() -> ()  [unwired: 1 in, 1 out]
          }
          event "Button.NextUnusedCtrls": Value Change {
            n77 = event-data() -> ()  [unwired: 1 in, 1 out]
          }
          event "VIs with Ctrl": Value Change {
            # "Will used by change the value of selected CTRL\nin the tab FP Translation .\nSee the case \"UI: FP Translation Update The Value ListOfVIs\"."
            n78 = event-data() -> ("NewVal"=w207:i32)  [unwired: 1 in]
            n79 = property on="VIs with Ctrl" class="LstBox (strict)"() -> ("Item Names"=w208:string[])  [unwired: 2 in, 2 out]
            n80 = Index Array(array=w208, index=w207) -> (element=w206:string)
            n81 = Bundle By Name(cluster=w214, "OldVal.ListOfVIs"=w206) -> (w209:T18)
            n82 = call <vilib>:"Add State(s) to Queue__JKI_lib_State_Machine.vi"("State(s) in (\"\")"=w210, "State(s) at Back (\"\")"="UI: FP Translation Show Control\nUI: FP Translation Update Control Visibility" ("State(s) at Back (\"\")")) -> ("States Out"=w211:string)  [unwired: 13 in]
          }
          event "Button.ZoomToCtrl": Value Change {
            n83 = event-data() -> ("NewVal"=w218:bool)  [unwired: 1 in]
            n84 = Select(t="UI: FP Translation Zoom To CTRL" ("State"), s=w218, f="UI: FP Translation Zoom Out" ("State")) -> (s? t:f=w216:string)
          }
          event "CTRL Index": Value Change {
            n85 = event-data() -> ()  [unwired: 1 in, 1 out]
            n86 = local read "Button.ZoomToCtrl"() -> (w227:bool)
            n87 = Select(t="UI: FP Translation Zoom To CTRL" ("State"), s=w227, f="UI: FP Translation Zoom Out" ("State")) -> (s? t:f=w224:string)
            n88 = call <vilib>:"Add State(s) to Queue__JKI_lib_State_Machine.vi"("State(s) in Front (\"\")"="UI: FP Translation Update Control Visibility" ("State(s) in Front (\"\")"), "State(s) in (\"\")"=w224) -> ("States Out"=w222:string)  [unwired: 13 in]
          }
          event "FP Translation Comment": Value Change {
            n89 = event-data() -> ()  [unwired: 1 in, 1 out]
          }
          event "Search Label": Value Change {
            n90 = event-data() -> ()  [unwired: 1 in, 1 out]
          }
          event "ListOfTextTranslations": Value Change {
            n91 = event-data() -> ()  [unwired: 1 in, 1 out]
          }
          event "AddTextToTranslate": Value Change {
            n92 = event-data() -> ()  [unwired: 1 in, 1 out]
          }
          event "DeleteText": Value Change {
            n93 = event-data() -> ()  [unwired: 1 in, 1 out]
          }
          event "TextTranslation": Value Change {
            n94 = event-data() -> ()  [unwired: 1 in, 1 out]
          }
          event "TT.TextANSI": Value Change {
            # "Delete NULL bytes from string.\nLabVIEW bug: Some times inserts LabVIEW NULL bytes by paste with Ctr-V."
            n95 = event-data() -> ("NewVal"=w256:string)  [unwired: 1 in]
            n96 = property on="TextTranslation" class="MCListbox (strict)"() -> ("ItemNames"=w263:string[][], "Value"=w261:i32)  [unwired: 2 in, 2 out]
            n97 = Search and Replace String(replace all?=TRUE ("replace all? (F)"), input string=w256, search string="\u0000") -> (result string=w255:string)  [unwired: 5 in, 3 out]
            n98 = Replace Array Subset(array=w263, new element=w255, index (row)=w261, index (col)=1 ("disabled index (col)")) -> (w262:string[][])
            n99 = local write "TT.TextANSI"(w255) -> ()
            n100 = property on="TextTranslation" class="MCListbox (strict)"("ItemNames"=w262) -> ()  [unwired: 2 in, 2 out]
          }
          event "TT.TextUnicode": Value Change {
            n101 = event-data() -> ("NewVal"=w269:string)  [unwired: 1 in]
            n102 = property on="TextTranslation" class="MCListbox (strict)"() -> ("ItemNames"=w273:string[][], "Value"=w271:i32)  [unwired: 2 in, 2 out]
            n103 = call "Add Unicode Header.vi"("Text"=w269) -> ("Text with header"=w268:string)  [unwired: 1 in, 1 out]
            n104 = Replace Array Subset(array=w273, new element=w268, index (row)=w271, index (col)=1 ("disabled index (col)")) -> (w272:string[][])
            n105 = property on="TextTranslation" class="MCListbox (strict)"("ItemNames"=w272) -> ()  [unwired: 2 in, 2 out]
          }
          event "TextName": Value Change {
            # "KEINE JKI-VIs, da sonst leerzeichen des NEW-Val gelöscht werden!"
            n106 = event-data() -> ("OldVal"=w277:string, "NewVal"=w279:string)  [unwired: 1 in]
            n107 = Format Into String(format string="Text Translation: Rename Text >> \"%s\" >> \"%s\"\nText Translation: Show Translation" ("State"), w277, w279) -> (resulting string=w278:string)  [unwired: 2 in, 1 out]
          }
          event "Save Settings": Value Change {
            n108 = event-data() -> ()  [unwired: 1 in, 1 out]
          }
          event "Controls": Value Change {
            # "Enable control if\nsome one contorl is added."
            n109 = event-data() -> ("NewVal"=w290:i32[])  [unwired: 1 in]
            n110 = for {
              tunnel: [w301] -> w291 mode=indexing
              tunnel: w290 -> [w300] mode=indexing
              tunnel: [w298] -> w289
              i -> [w297]
              w296 = T4."Disabled and Grayed Out" ("Disabled")
              n111 = property on="Controls" class="MCListbox (strict)"() -> ("ItemNames"=w305:string[][])  [unwired: 2 in, 2 out]
              n112 = Index Array(array=w305, index (row)=w300, index (col)=3 ("disabled index (col)")) -> (element=w303:string)
              n113 = Not Equal?(x=w303, y="Not Added") -> (x != y?=w299:bool)
              n114 = case shown="0" w297 {
                tunnel: w299 -> [_ w310]
                tunnel: w296 -> [w306 w309]
                tunnel: [w306 w307] -> w298
                frame Default {
                }
                frame 0 {
                  n115 = Select(t=T4."Enabled", s=w310, f=w309) -> (s? t:f=w307:T4)
                }
              }
              n116 = Select(t=w296, s=w299, f=T4."Enabled" ("Disabled")) -> (s? t:f=w301:T4)
            }
            n117 = Array Max & Min(array=w291) -> (min value=w288:T4)  [unwired: 3 out]
            n118 = property on="Button.AddToFPTranslation" class="Bool"("DisabledEnum"=w288) -> ()  [unwired: 2 in, 2 out]
            n119 = property on="Button.GoToTranslation" class="Bool"("DisabledEnum"=w289) -> ()  [unwired: 2 in, 2 out]
          }
          event "Button.GoToTranslation": Value Change {
            # "Das gesuchte ist mit dem Search Label immer oben"
            # "Damit links das korrekte angezeigt wird.\nArbeite mit Filter als schnelle Lösung!"
            # "Activaze the tab \"Front Panel ranslation\""
            # "Get label name"
            n120 = event-data() -> ()  [unwired: 1 in, 1 out]
            n121 = property on="Controls" class="MCListbox (strict)"() -> ("ItemNames"=w320:string[][], "Value"=w319:i32[])  [unwired: 2 in, 2 out]
            n122 = Index Array(array=w319) -> (element=w321:i32)  [unwired: 1 in]
            n123 = Index Array(array=w320, index (row)=w321, index (col)=0 ("disabled index (col)")) -> (element=w315:string)
            n124 = local write "Tab Control"(T1."Front Panel Translation" ("Tab Control")) -> ()
            n125 = local write "ListOfControls"(0 ("ListOfControls")) -> ()
            n126 = local write "Search Label"(w315) -> ()
            n127 = call <vilib>:"Build State String with Arguments__JKI_lib_State_Machine.vi"("Arguments (\"\")"=w315, "State"="Macro: List Of Controls Value Change") -> ("State with Arguments"=w312:string)  [unwired: 4 in]
            n128 = call <vilib>:"Add State(s) to Queue__jki_lib_state_machine.vi"("State(s) in (\"\")"="UI: FP Translation Filter ListOfControls" ("f"), "State(s) at Back (\"\")"=w312) -> ("States Out"=w314:string)  [unwired: 13 in]
          }
          event "VIs": Double Click {
            n129 = event-data() -> ()  [unwired: 1 in, 1 out]
          }
          event "Search text": Value Change {
            n130 = event-data() -> ()  [unwired: 1 in, 1 out]
          }
          event "DelFilter": Value Change {
            n131 = event-data() -> ()  [unwired: 1 in, 1 out]
            n132 = property on="Search Label" class="Str"("Val(Sgnl)"="") -> ()  [unwired: 2 in, 2 out]
          }
          event "Language Config Path": Value Change {
            n133 = event-data() -> ()  [unwired: 1 in, 1 out]
            n134 = call <vilib>:"Is Path and Not Empty.vi"("path"="Language Config Path") -> ("Is Path and Not Empty?"=w340:bool)  [unwired: 4 in]
            n135 = Select(t="Macro: Read Translation File" ("State with Arguments"), s=w340, f="") -> (s? t:f=w338:string)
          }
          event "Export to txt": Value Change {
            n136 = event-data() -> ()  [unwired: 1 in, 6 out]
            n137 = One Button Dialog(message="Note:\nWhen opening the exported Unicode files in a text editor, special characters appear at the end of each line.") -> ()  [unwired: 1 in, 1 out]
          }
          event "Import": Value Change {
            n138 = event-data() -> ()  [unwired: 1 in, 1 out]
            n139 = call "File Dialog2"("error in"=w351) -> ("selected path"=w354:path, "cancelled"=w353:bool, "error out"=w352:errorcluster)  [unwired: 11 in, 1 out]
            n140 = case shown="False" w353 {
              tunnel: [w360 _] -> w355
              tunnel: w354 -> [w359 _]
              frame False {
                n141 = Path To String(path=w359) -> (string=w358:string)
                n142 = call <vilib>:"Build State String with Arguments__JKI_lib_State_Machine.vi"("Arguments (\"\")"=w358, "State"="Macro: Import Translations" ("f")) -> ("State with Arguments"=w360:string)  [unwired: 4 in]
              }
              frame True {
              }
            }
            n143 = call <vilib>:"Clear Errors.vi"("error in (no error)"=w352) -> ("error out"=w350:errorcluster)  [unwired: 5 in, 1 out]
          }
        }
        n144 = call <vilib>:"Add State(s) to Queue__JKI_lib_State_Machine.vi"("State(s) in (\"\")"=w16, "State(s) at Back (\"\")"=w17) -> ("States Out"=w18:string)  [unwired: 13 in]
      }
      frame Error {
        # "Errors we be handled first."
      }
    }
    n145 = while {
      tunnel: [w376] -> w10
      tunnel: [w372] -> w5
      shift-right: [w370] -> w7
      shift-left: w11 -> [w377]
      shift-right: [w366] -> w14
      shift-left: w9 -> [w375]
      shift-right: [w379] -> w15
      shift-left: w12 -> [w378]
      stop <- w367 stop-if-true
      n146 = call <vilib>:"Parse State Queue__JKI_lib_State_Machine.vi"("State Queue"=w377, "Error In (no error)"=w375) -> ("Remaining States"=w374:string, "Current State"=w365:string, "Arguments"=w373:string)  [unwired: 11 in]
      n147 = case shown="\"Data: Init with Import\"" w365 {
        selector: w365 -> [_ w389 _ _ _ _ _ _ _ _ _ _ _ _ _ _ _ _ _ _ _ _ _ _ _ _ _ _ _ _ _ _ _ _ _ _ _ _ _ _ _ _ _ _ _ _ _ _ _ _ _ _ _ _ _ _ _ _ _ _ _ _ _ _ _]
        tunnel: w374 -> [w386 w395 w407 w410 w416 w419 w421 w435 w451 w478 w485 w498 w532 w539 w563 w564 w569 w597 w603 w659 w678 w686 w700 w750 w775 w803 w838 w858 w871 w883 w932 w938 w945 w960 w963 w967 w974 w985 w991 w997 w1007 w1028 w1064 w1066 w1126 w1153 w1163 w1168 w1212 w1223 w1228 w1248 w1250 w1262 w1274 w1290 w1316 w1326 w1335 w1363 w1369 w1388 w1399 w1428 w1446]
        tunnel: w373 -> [_ _ _ _ _ _ _ _ _ w452 _ _ _ _ _ _ _ w590 _ _ _ _ _ _ w770 w798 w833 _ _ _ _ _ _ _ _ _ w971 w977 _ _ _ _ _ _ _ _ _ _ _ _ _ _ w1251 _ w1275 _ _ _ _ _ w1370 _ w1400 _ _]
        tunnel: w378 -> [w382 w396 w398 w409 w415 w418 w422 _ w449 w476 w482 w500 w530 w542 w561 w565 w568 w596 w602 w660 w670 w685 w709 w737 w781 w804 w839 w859 w869 w885 w933 w936 w944 w961 w964 w968 w975 w986 w993 w998 w1006 w1027 w1063 w1068 w1128 w1150 w1162 w1170 w1211 w1222 w1238 w1247 w1253 w1261 w1277 w1289 w1302 w1325 w1349 w1362 w1372 w1390 w1402 w1430 w1450]
        tunnel: [w385 w388 w408 w411 errorcluster {"status"=FALSE, "code"=0, "source"=""} ("error out") w420 w423 w436 w438 w462 w483 w499 w531 w546 w560 w566 w567 w598 w601 w662 w679 w687 w710 w751 w782 w802 w837 w857 w870 w884 w926 w937 w946 w962 w965 w969 w976 w987 w996 w999 w1001 w1025 w1065 w1069 w1129 w1154 w1164 w1166 w1213 w1224 w1229 w1249 w1254 w1263 w1278 w1292 w1317 w1327 w1350 w1364 w1373 w1391 w1403 w1432 w1453] -> w366
        tunnel: w375 -> [w385 w387 w408 w411 w414 w420 w423 w436 w450 w477 w484 w497 w531 w546 w559 w566 w567 w598 w601 w662 w679 w687 w710 w751 w784 w802 w837 w857 w870 w884 w927 w937 w943 w962 w965 w969 w976 w987 w996 w999 w1002 w1016 w1065 w1069 w1129 w1154 w1164 w1167 w1213 w1224 w1230 w1249 w1254 w1263 w1278 w1292 w1317 w1327 w1350 w1364 w1373 w1391 w1403 w1432 w1453]
        tunnel: [w386 w395 w407 w410 w416 w419 w421 w435 w451 w478 w485 w498 w532 w539 w563 w564 w569 w597 w603 w659 w678 w686 w700 w750 w775 w803 w838 w858 w871 w883 w932 w938 w945 w960 w963 w967 w974 w985 w991 w997 w1007 w1028 w1064 w1066 w1126 w1153 w1163 w1168 w1212 w1223 w1228 w1248 w1250 w1262 w1274 w1290 w1316 w1326 w1335 w1363 w1369 w1388 w1399 w1428 w1446] -> w371
        tunnel: [w382 w396 w397 w409 w415 w418 w422 w434 w445 w472 w482 w501 w529 w543 w561 w565 w568 w596 w602 w660 w670 w685 w709 w737 w776 w804 w839 w859 w869 w878 w933 w936 w944 w961 w964 w968 w975 w986 w993 w998 w1006 w1027 w1063 w1067 w1127 w1150 w1162 w1169 w1210 w1221 w1238 w1247 w1252 w1260 w1276 w1291 w1302 w1325 w1349 w1362 w1371 w1389 w1401 w1431 w1450] -> w379
        tunnel: [_ _ _ _ _ w417 _ _ _ _ _ _ _ _ _ _ _ _ _ _ _ _ _ _ _ _ _ _ _ _ _ _ _ _ _ _ _ _ _ _ _ _ _ _ _ _ _ _ _ _ _ _ _ _ _ _ _ _ _ _ _ _ _ _ _] -> w376
        tunnel: [-1 _ _ _ _ _ _ _ _ _ _ _ _ _ _ _ _ _ _ _ _ _ _ _ _ _ _ _ _ _ _ _ _ _ _ _ _ _ _ _ _ _ _ _ _ _ _ _ _ _ _ _ _ _ _ _ _ _ _ _ _ _ _ _ _] -> w372
        tunnel: ["/* States to execute repeatedly if idle" _ _ _ "/* Post Error States" _ _ _ _ _ _ _ _ _ _ _ _ _ _ _ _ _ _ _ _ _ _ _ _ _ _ _ _ _ _ _ _ _ _ _ _ _ _ _ _ _ _ _ _ _ _ _ _ _ _ _ _ _ _ _ _ _ _ _ _] -> w369
        tunnel: ["" _ _ _ _ _ _ _ w440 w466 _ _ _ _ _ _ _ _ _ _ _ _ _ _ _ _ _ _ _ _ _ _ _ _ "Initialize Core Data\nUI: Initialize\nUI: Enable Controls >> False\nLanguages: Search" "Data: Initialize\nData: Get VIs Controls\nUI: List Of Controls Update\nUI: File Changed" w973 w978 w992 _ _ _ _ _ _ _ _ _ _ _ _ _ _ _ _ _ _ _ _ _ _ _ _ _ _] -> w368
        tunnel: [TRUE _ _ _ _ w417 _ _ _ _ _ _ _ _ _ _ _ _ _ _ _ _ _ _ _ _ _ _ _ _ _ _ _ _ _ _ _ _ _ _ _ _ _ _ _ _ _ _ _ _ _ _ _ _ _ _ _ _ _ _ _ _ _ _ _] -> w367
        frame "", "Idle" {
          # "After this Idle-Case, we quit this inner while loop to check the event-structure for new User-Events"
          # "executes when the state queue is empty"
        }
        frame Default {
          w393 = 42 items=["No error", "Argument error", "Memory is full", "Out of zone", "End of file", "File already open", "Generic file I/O error", "File not found", "File permission error", "Disk is full", "Duplicate path", "Too many files open", "System feature not enabled", "Resource file not found", "Cannot add resource", "Resource not found", "Image not found", "Image memory error", "Pen does not exist", "Config type invalid", "Config token not found", "Config parse error", "Config memory error", "Bad external code format", "Bad external code offset", "External code not present", "Null window", "Destroy window error", "Null menu", "Print aborted", "Bad print record", "Print driver error", "Windows error during printing", "Memory error during printing", "Print dialog error", "Generic print error", "Invalid device refnum", "Device not found", "Device parameter error", "Device unit error", "Cannot open device", "Device call aborted", "Generic error", "Cancelled by user", "Object ID too low", "Object ID too high", "Object not in heap", "Unknown heap", "Unknown object (invalid DefProc)", "Unknown object (DefProc not in table)", "Message out of range", "Invalid (null) method", "Unknown message", "Manager call not supported", "Bad address", "Network operation in progress", "Network operation timed out", "Connection is busy", "Network attribute not supported", "Network error", "Address in use", "System out of memory", "Connection aborted", "Connection refused", "Not connected", "Already connected", "Connection closed", "Initialization error (interapplication manager)", "Bad occurrence", "Wait on unbound occurrence handler", "Occurrence queue overflow", "Datalog type conflict", "Unused", "Unrecognized type (interapplication manager)", "Memory corrupt", "Failed to make temporary DLL", "Old CIN version", "Drag socket not found", "Failed to load drop-object", "Failed to register OLE object", "Failed to release OLE object", "Format specifier type mismatch", "Unknown format specifier", "Too few format specifiers", "Too many format specifiers", "Scan failed", "Newer CIN version", "Error converting to variant", "Runtime menu error", "Password tampered", "Variant attribute not found", "Incompatible variant data type", "Event data is not available", "Event Store is not present", "Occurrence is not found", "Event Queue is not created", "Event info is not available", "Refnum passed is NULL", "Error retrieving Class GUID", "Error retrieving CoClass GUID", "Error retrieving TypeLib GUID.", "Bad built application magic bytes.", "Specific driver is different from the specific driver associated with the Logical Name.", "There is no session opened to the class driver.", "Max Error", "MAX - Error with config objects", "MAX - Error loading configuration", "MAX - Group not supported"]
          # "Handle mistyped state name (developer tool)"
          # "Do not delete, rename, or modify this frame.\n(this is used to capture unhandled states and typos)"
          n148 = Format Into String(format string="Software Exception: Unhandled State \"%s\"." ("message"), error in=w387, w389) -> (resulting string=w392:string, error out=w391:errorcluster)  [unwired: 1 in]
          n149 = call <vilib>:"Error Cluster From Error Code.vi"("show call chain? (False)"=TRUE, "error in (no error)"=w391, "error message (\"\")"=w392, "error code (0)"=w393) -> ("error out"=w388:errorcluster)  [unwired: 5 in]
        }
        frame "Initialize Core Data" {
          # "originally closed?"
          # "exe?"
          # "If panel starts closed or is an EXE, then close it when we exit"
          n150 = property class="VI"() -> ("FP.State"=w405:T5)  [unwired: 2 in, 2 out]
          n151 = property class="App"() -> ("App.Kind"=w401:T6)  [unwired: 2 in, 2 out]
          n152 = control-ref of="Current VI Reference"() -> (w404:refnum<vi>)
          n153 = Equal?(x=w405, y=T5."Closed" ("Front Panel Window:State")) -> (x = y?=w406:bool)
          n154 = Equal?(x=w401, y=T6."Run Time System" ("Application:Kind")) -> (x = y?=w402:bool)
          n155 = Or(x=w406, y=w402) -> (x .or. y?=w403:bool)
          n156 = Bundle By Name(cluster=w398, "Core.Current VI Reference"=w404, "Core.Close Panel on Exit?"=w403) -> (w397:T18)
        }
        frame "Release Core Data" {
        }
        frame "Error Handler" {
          # "Unhandled Error -- Display it"
          # "Clear error"
          n157 = call <vilib>:"General Error Handler.vi"("error in (no error)"=w414) -> ()  [unwired: 10 in, 5 out]
        }
        frame "Exit" {
          w417 = TRUE ("Exit?")
          # "Do not put any code in this frame.\n(No errors that occur here will be handled.)"
        }
        frame "---------- Data ----------" {
          # "Do not put any code in this frame.\n(It is a separator no-op. You can make a copy of this frame to create a new Data frame)"
        }
        frame "Data Cluster" {
          w424 = T19 {"Current VI Reference"=refnum, "Close Panel on Exit?"=FALSE}  # Core
          w425 = T10 {"Horizontal"=0, "Vertical"=0}  # Origin
          w426 = map{string, T14} {}  # T.Tr
          w427 = map{string, T14} {}  # FP.Tr
          w428 = 1.0  # ZoomOutFactor
          w429 = ""  # OldVal.ListOfVIs
          w430 = T17[] []  # Selected CTRLs
          w431 = T20 {"Item Names"=[], "Item Symbols"=[]}  # Controls
          w432 = map{path, T17[]} {}  # CTRLs
          w433 = T15 {"Data"={"Startup Language"="", "Default Language"="", "Languages"={"ANSI"=[], "Unicode"=[]}}, "Supported Languages"={"ANSI"=[], "Unicode"=[]}, "VIs"=[], "FP Translations"=[], "Text Translations"=[]}  # LT
          # "This Case does not have to execute. It is ment to define the data structure of the actor´s data cluster.\n(data names are defined by what you wire into the bundle function)"
          n158 = Bundle("Core"=w424, "LT"=w433, "CTRLs"=w432, "Controls"=w431, "Selected CTRLs"=w430, "OldVal.ListOfVIs"=w429, "ZoomOutFactor"=w428, "FP.Tr"=w427, "T.Tr"=w426, "Origin"=w425) -> (w434:T18)  [unwired: 1 in]
        }
        frame "Data: Initialize" {
          # "Creates the list of controls.\nThis array is unfiltered list of controls, that supports the viewing of the List of controls on the tab \"Front Panel Translation\"."
          # "Initialize the shift-register data, here. do not delete - used by framework"
          n159 = local read "Language Config Path"() -> (w442:path)
          n160 = call "Read Language Selection UTF-16 LE.vi"("error in (no error)"=w450, "LanguageSelection file"=w442) -> ("error out"=w438:errorcluster, "Language Selection"=w443:T15)  [unwired: 8 in]
          n161 = Bundle By Name(cluster=w449, "LT"=w443) -> (w446:T18)
          n162 = Unbundle By Name(w446) -> ("LT.FP Translations"=w448:T7[], "LT.Text Translations"=w447:T7[])
          n163 = Not(x=w438) -> (.not. x?=w437:bool)
          n164 = call "Create Map from Translations.vi"("Translations"=w448) -> ("Map out"=w441:map{string, T14})
          n165 = call "Create Map from Translations.vi"("Translations"=w447) -> ("Map out"=w444:map{string, T14})
          n166 = Format Into String(format string="UI: Enable Controls >> %s" ("States Out"), w437) -> (resulting string=w440:string)  [unwired: 2 in, 1 out]
          n167 = Bundle By Name(cluster=w446, "FP.Tr"=w441, "T.Tr"=w444) -> (w445:T18)
        }
        frame "Data: Init with Import" {
          # "Initialize the shift-register data, here. do not delete - used by framework"
          n168 = local read "Language Config Path"() -> (w463:path)
          n169 = call "Read Language Selection UTF-16 LE.vi"("error in (no error)"=w477, "LanguageSelection file"=w463) -> ("error out"=w461:errorcluster, "Language Selection"=w470:T15)  [unwired: 8 in]
          n170 = call <vilib>:"Get File Extension.vi"("file"=w463) -> ("filename without extension"=w459:string)  [unwired: 6 in, 4 out]
          n171 = Format Into String(format string="%s\\\\%s_Text_ansi.txt", w452, w459) -> (resulting string=w457:string)  [unwired: 2 in, 1 out]
          n172 = Format Into String(format string="%s\\\\%s_Frontpanel_ansi.txt", w452, w459) -> (resulting string=w455:string)  [unwired: 2 in, 1 out]
          n173 = String To Path(string=w457) -> (path=w456:path)
          n174 = String To Path(string=w455) -> (path=w454:path)
          n175 = call "Import from text file.vi"("error in (no error)"=w461, "File to import"=w454) -> ("error out"=w458:errorcluster, "Text Translations"=w453:T7[])  [unwired: 8 in]
          n176 = call "Import from text file.vi"("error in (no error)"=w458, "File to import"=w456) -> ("error out"=w462:errorcluster, "Text Translations"=w465:T7[])  [unwired: 8 in]
          n177 = Bundle By Name(cluster=w476, "LT"=w470, "LT.FP Translations"=w453, "LT.Text Translations"=w465) -> (w473:T18)
          n178 = Not(x=w462) -> (.not. x?=w467:bool)
          n179 = Unbundle By Name(w473) -> ("LT.FP Translations"=w475:T7[], "LT.Text Translations"=w474:T7[])
          n180 = call "Create Map from Translations.vi"("Translations"=w475) -> ("Map out"=w469:map{string, T14})
          n181 = call "Create Map from Translations.vi"("Translations"=w474) -> ("Map out"=w471:map{string, T14})
          n182 = Format Into String(format string="UI: Enable Controls >> %s" ("States Out"), w467) -> (resulting string=w466:string)  [unwired: 2 in, 1 out]
          n183 = Bundle By Name(cluster=w473, "FP.Tr"=w469, "T.Tr"=w471) -> (w472:T18)
        }
        frame "Data: Save" {
          n184 = Unbundle By Name(w482) -> ("LT"=w481:T15)
          n185 = local read "Language Config Path"() -> (w480:path)
          n186 = call <vilib>:"Is Path and Not Empty.vi"("path"=w480) -> ("Is Path and Not Empty?"=w479:bool)  [unwired: 4 in]
          n187 = case shown="True" w479 {
            tunnel: w484 -> [w486 w490]
            tunnel: [w486 w489] -> w483
            tunnel: w481 -> [_ w488]
            tunnel: w480 -> [_ w487]
            frame False {
            }
            frame True {
              n188 = call "Write Language Selection UTF-16 LE.vi"("error in (no error)"=w490, "Langúage Selection"=w488, "LanguageSelection file"=w487) -> ("error out"=w489:errorcluster)  [unwired: 7 in, 1 out]
            }
          }
        }
        frame "Data: Get VIs Controls" {
          n189 = local read "App File Path"() -> (w492:path)
          n190 = Unbundle By Name(w500) -> ("LT.VIs"=w496:path[])
          n191 = disable-structure shown="Default" {
            disable-tunnel: w497 -> [w503 w514]
            disable-tunnel: w496 -> [w505 w513]
            disable-tunnel: [w503 w512] -> w495
            disable-tunnel: [w505 w511] -> w494
            disable-tunnel: [w504 w510] -> w493
            disable-tunnel: w492 -> [w502 _]
            disable-tunnel: "Top Level VI" -> [_ w509]
            frame condition #0 (active) {
              n192 = for {
                tunnel: w505 -> [w508] mode=indexing
                tunnel: [w507] -> w504 mode=indexing
                tunnel: w502 -> [w506]
                n193 = Build Path(base path=w506, name or relative path=w508) -> (appended path=w507:path)
              }
            }
            frame condition #1 {
              n194 = call "Get VI Refs To Translate.vi"("error in (no error)"=w514, "Top Level VI"=w509, "Expected VIs"=w513) -> ("error out"=w512:errorcluster, "VIs"=w510:path[], "VIs Relative Path"=w511:path[])  [unwired: 5 in, 1 out]
            }
          }
          n195 = in-place {
            in-place-border: w494 -> [w517]
            in-place-border: w495 -> [w519]
            in-place-border: [w515] -> w499
            in-place-border: w493 -> [w516]
            n196 = in-place-cluster #1(w500) -> ("CTRLs"=w521:map{path, T17[]})
            n197 = for {
              tunnel: w517 -> [w523] mode=indexing
              shift-right: [w527] -> w520
              shift-left: w521 -> [w528]
              tunnel: w516 -> [w522] mode=indexing
              tunnel: w519 -> [w525]
              tunnel: [w524] -> w518 mode=indexing
              n198 = call "Get All Controls.vi"("error in (no error)"=w525, "VI"=w522) -> ("error out"=w524:errorcluster, "VIs Controls"=w526:T17[])  [unwired: 8 in]
              n199 = Insert Into Map(map in=w528, key=w523, value=w526) -> (map out=w527:map{path, T17[]})  [unwired: 2 out]
            }
            n200 = in-place-cluster #1("CTRLs"=w520) -> (w501:T18)
            n201 = Merge Errors(w518) -> (w515:errorcluster)
          }
        }
        frame "Data: FP Translation Edit Comment" {
          n202 = in-place {
            n203 = in-place-cluster #2(w530) -> ("FP.Tr"=w535:map{string, T14})
            n204 = local read "Label"() -> (w534:string)
            n205 = in-place {
              n206 = in-place-map #3(w535, w534) -> (w538:T14)  [unwired: 1 in, 1 out]
              n207 = Bundle By Name(cluster=w538, "Comment"="FP Translation Comment") -> (w537:T14)
              n208 = in-place-map #3(w537) -> (w533:map{string, T14})  [unwired: 1 in, 2 out]
            }
            n209 = in-place-cluster #2("FP.Tr"=w533) -> (w529:T18)
          }
        }
        frame "Data: Update Config" {
          # "Get labels"
          n210 = Unbundle By Name(w542) -> ("FP.Tr"=w541:map{string, T14}, "T.Tr"=w540:map{string, T14})
          n211 = for {
            tunnel: w540 -> [w549] mode=indexing
            tunnel: [w548] -> w544 mode=indexing
            n212 = Unbundle By Name(w549) -> ("Translation.Comment"=w551:string, "Translation.Properties"=w550:T8[], "Label"=w547:string)
            n213 = Bundle By Name(cluster=T7 {"Label"="", "Comment"="", "Property"=[]} ("Control"), "Comment"=w551, "Property"=w550, "Label"=w547) -> (w548:T7)
          }
          n214 = for {
            tunnel: w541 -> [w554] mode=indexing
            tunnel: [w555] -> w545 mode=indexing
            n215 = Unbundle By Name(w554) -> ("Translation.Comment"=w557:string, "Translation.Properties"=w556:T8[], "Label"=w553:string)
            n216 = Bundle By Name(cluster=T7 {"Label"="", "Comment"="", "Property"=[]} ("Control"), "Comment"=w557, "Property"=w556, "Label"=w553) -> (w555:T7)
          }
          n217 = Bundle By Name(cluster=w542, "LT.FP Translations"=w545, "LT.Text Translations"=w544) -> (w543:T18)
        }
        frame "Data: Cleanup" {
          # "Cleanup any data and references, here.\n(this is called automatically, by the Macro: Exit)"
          n218 = Unbundle By Name(w561) -> ("Core.Current VI Reference"=w562:refnum<vi>)
          n219 = Close Reference(reference=w562, error in (no error)=w559) -> (error out=w560:errorcluster)
        }
        frame "---------- UI ----------" {
          # "Do not put any code in this frame.\n(It is a separator no-op. You can make a copy of this frame to create a new UI frame)"
        }
        frame "UI: Initialize" {
          # "Initialize the User Interface, here.\n(this is called automatically, by the Macro: Init)"
          n220 = stacked-sequence {
            frame #0 {
              w571 = 0
              # "If Actor is running standalone show the Init and Exit Buttons"
              # "General"
              n221 = disable-structure shown="RUN_TIME_ENGINE==True" {
                disable-tunnel: [TRUE _] -> w574
                frame condition #0 (active) {
                }
                frame condition #1 {
                }
              }
              n222 = call <vilib>:"Application Directory.vi"() -> ("Application Directory"=w572:path)
              n223 = local write "Language Config Path"(path "" ("Language Config Path")) -> ()
              n224 = local write "App File Path"(w572) -> ()
              n225 = property on="Init" class="Bool"("Visible"=w574) -> (error out=w579:errorcluster)  [unwired: 2 in, 1 out]
              n226 = property on="AddCtrlToTranslate" class="Bool"("Visible"=w574) -> ()  [unwired: 2 in, 2 out]
              n227 = property on="Tab Control" class="TabCtl (strict)"() -> ("Pages"=w575:refnum<vi>[])  [unwired: 2 in, 2 out]
              n228 = property on="Exit" class="Bool"(error in=w579, "Visible"=w574) -> ()  [unwired: 1 in, 2 out]
              n229 = Index Array(array=w575, index=2) -> (element=w578:refnum<vi>)
              n230 = property on="DelCtrlToTranslate" class="Bool"("Visible"=w574) -> ()  [unwired: 2 in, 2 out]
              n231 = property class="Page"(reference=w578, "PageVis"=w574) -> (error out=w576:errorcluster)  [unwired: 1 in, 1 out]
              n232 = property on="Class Name" class="Enum (strict)"("Visible"=w574) -> ()  [unwired: 2 in, 2 out]
              n233 = property on="Pane" class="Pane"("Origin"=T10 {"Horizontal"=0, "Vertical"=0}) -> ()  [unwired: 2 in, 2 out]
              n234 = local write "Tab Control"(w571) -> ()
              n235 = Close Reference(reference=w575, error in (no error)=w576) -> ()  [unwired: 1 out]
              n236 = local write "TextTranslation"(w571) -> ()
              n237 = property on="Button.NextUnusedCtrls" class="Bool"("Visible"=w574) -> ()  [unwired: 2 in, 2 out]
              n238 = local write "Search"("" ("Search")) -> ()
            }
            frame #1 {
              w585 = -1 ("ListOfControls")
              w586 = string[][] [] ("Item Names")
              n239 = property on="Controls" class="MCListbox (strict)"("ItemNames"=w586, "Value"=i32[] [] ("Controls")) -> ()  [unwired: 2 in, 2 out]
              n240 = property on="VIs" class="MCListbox (strict)"("ItemNames"=w586, "Value"=-1 ("VIs")) -> ()  [unwired: 2 in, 2 out]
              n241 = property on="ListOfTextTranslations" class="LstBox (strict)"("Item Names"=string[] [], "Value"=w585) -> ()  [unwired: 2 in, 2 out]
              n242 = property on="TextTranslation" class="MCListbox (strict)"("ItemNames"=w586, "Value"=w585) -> ()  [unwired: 2 in, 2 out]
              n243 = property on="ListOfControls" class="MCListbox (strict)"("ItemNames"=w586, "Val(Sgnl)"=w585) -> ()  [unwired: 2 in, 2 out]
            }
          }
        }
        frame "UI: Enable Controls" {
          n244 = control-ref of="Tab Control"() -> (w595:refnum<vi>)
          n245 = control-ref of="Import"() -> (w587:refnum<vi>)
          n246 = control-ref of="Save"() -> (w593:refnum<vi>)
          n247 = control-ref of="Save As"() -> (w592:refnum<vi>)
          n248 = control-ref of="Export to txt"() -> (w591:refnum<vi>)
          n249 = Build Array(w595, w593, w592, w591, w587) -> (w594:refnum<vi>[])
          n250 = Scan From String(input string=w590, default 1=FALSE) -> (output 1=w588:bool)  [unwired: 3 in, 3 out]
          n251 = for {
            tunnel: w588 -> [w600]
            tunnel: w594 -> [w599] mode=indexing
            n252 = call <vilib>:"Enable or Gray Control Refnum.vi"("enable?"=w600, "Control in"=w599) -> ()  [unwired: 8 in, 2 out]
          }
        }
        frame "UI: File Changed" {
          # "Initialize the User Interface, here.\n(this is called automatically, by the Macro: Init)"
          n253 = stacked-sequence {
            tunnel: w602 -> [w612 w619 _ w651]
            frame #0 {
              # "The default language can only be ASCII, because that is used for the properties that do not support Unicode."
              # "Languages"
              n254 = Unbundle By Name(w612) -> ("LT.Data.Languages.ANSI"=w604:string[], "LT.Data.Languages.Unicode"=w613:string[], "LT.Data.Startup Language"=w610:string, "LT.Data.Default Language"=w611:string)
              n255 = local write "ControlsFilter"(T2 {"VI.Filter.Label"="", "VI.Filter.Class"="", "No Error Cluster"=TRUE, "NonTranslated"=FALSE, "OnlyVisibleArea"=TRUE} ("ControlsFilter")) -> ()
              n256 = local write "AllLanguages"(-1 ("AllLanguages")) -> ()
              n257 = property on="Delete" class="Bool"("DisabledEnum"=T4."Disabled and Grayed Out" ("Disabled")) -> ()  [unwired: 2 in, 2 out]
              n258 = Build Array (concatenate)(w604, w613) -> (w609:string[])
              n259 = property on="StartLang" class="CmbBox"("Strings[]"=w609, "Value"=w610) -> ()  [unwired: 2 in, 2 out]
              n260 = property on="DefLang" class="CmbBox"("Strings[]"=w604, "Value"=w611) -> ()  [unwired: 2 in, 2 out]
              n261 = property on="Languages" class="LstBox (strict)"("Item Names"=w609, "Value"=-1 ("Languages")) -> ()  [unwired: 2 in, 2 out]
            }
            frame #1 {
              w616 = T4."Disabled and Grayed Out" ("Disabled")
              # "VIs"
              n262 = local read "App File Path"() -> (w614:path)
              n263 = Unbundle By Name(w619) -> ("LT.VIs"=w622:path[])
              n264 = for {
                tunnel: w622 -> [w626] mode=indexing
                tunnel: [w625] -> w623 mode=indexing
                n265 = Strip Path(path=w626) -> (name=w625:string)  [unwired: 1 out]
              }
              n266 = property on="Controls" class="MCListbox (strict)"("ItemNames"=string[][] [] ("Item Names"), "Value"=i32[] [] ("Controls")) -> ()  [unwired: 2 in, 2 out]
              n267 = call "Get VI library name.vi"("App File Path"=w614, "VIs"=w622) -> ("Library or Error String"=w621:string[])  [unwired: 8 in, 1 out]
              n268 = Build Array(w623, w621) -> (w624:string[][])
              n269 = property on="Button.AddToFPTranslation" class="Bool"("DisabledEnum"=w616) -> ()  [unwired: 2 in, 2 out]
              n270 = property on="Button.GoToTranslation" class="Bool"("DisabledEnum"=w616) -> ()  [unwired: 2 in, 2 out]
              n271 = Transpose 2D Array(2D array=w624) -> (transposed array=w620:string[][])
              n272 = property on="VIs" class="MCListbox (strict)"("ItemNames"=w620, "Value"=-1 ("VIs")) -> ()  [unwired: 2 in, 2 out]
            }
            frame #2 {
              w631 = ""
              # "Fornt Panel Translation"
              n273 = invoke on="Tree" class="Tree (strict)" method="Edit Tree Items.Delete"("Delete Children"=TRUE ("Delete Children?")) -> ()  [unwired: 4 in, 5 out]
              n274 = control-ref of="FPT.TextUnicode"() -> (w630:refnum<vi>)
              n275 = call <vilib>:"Property Interpret As Unicode.vi"("Interpret As Unicode (T)"=TRUE, "String Control Reference"=w630) -> ("error out"=w628:errorcluster, "String Control Reference"=w629:refnum<vi>)  [unwired: 6 in]
              n276 = Close Reference(reference=w629, error in (no error)=w628) -> ()  [unwired: 1 out]
              n277 = local write "FPT.TextUnicode"(w631) -> ()
              n278 = local write "FPT.TextANSI"(w631) -> ()
            }
            frame #3 {
              w641 = ""
              # "Diese Übersetzungen haben einen extra Case, der vorher aufgerufen wird!"
              # "Text Translations"
              n279 = Unbundle By Name(w651) -> ("T.Tr"=w650:map{string, T14}, "LT.Data.Languages.ANSI"=w647:string[], "LT.Data.Languages.Unicode"=w646:string[])
              n280 = control-ref of="TT.TextUnicode"() -> (w637:refnum<vi>)
              n281 = local write "FP Translation Comment"(w641) -> ()
              n282 = local write "Button.ZoomToCtrl"(FALSE ("Button.ZoomToCtrl")) -> ()
              n283 = local write "Tree"(w641) -> ()
              n284 = call <vilib>:"Property Interpret As Unicode.vi"("Interpret As Unicode (T)"=TRUE, "String Control Reference"=w637) -> ("error out"=w634:errorcluster, "String Control Reference"=w635:refnum<vi>)  [unwired: 6 in]
              n285 = for {
                tunnel: w650 -> [w653] mode=indexing
                tunnel: [w652] -> w649 mode=indexing
                n286 = Unbundle By Name(w653) -> ("Label"=w652:string)
              }
              n287 = Build Array("") -> (w639:string[])
              n288 = Build Array (concatenate)(w647, w646) -> (w645:string[])
              n289 = Close Reference(reference=w635, error in (no error)=w634) -> ()  [unwired: 1 out]
              n290 = Build Array(w645, w639) -> (w644:string[][])
              n291 = Transpose 2D Array(2D array=w644) -> (transposed array=w643:string[][])
              n292 = property on="ListOfTextTranslations" class="LstBox (strict)"("Item Names"=w649, "Value"=-1 ("ListOfTextTranslations")) -> ()  [unwired: 2 in, 2 out]
              n293 = property on="TextTranslation" class="MCListbox (strict)"("ItemNames"=w643, "Value"=-1 ("TextTranslation")) -> ()  [unwired: 2 in, 2 out]
              n294 = property on="ListOfControls" class="MCListbox (strict)"("Val(Sgnl)"=-1 ("ListOfControls")) -> ()  [unwired: 2 in, 2 out]
            }
          }
        }
        frame "UI: Languages" {
          # "For update TT tab."
          # "For update FPT tab."
          n295 = Unbundle By Name(w660) -> ("LT.Data.Default Language"=w656:string, "LT.Data.Languages.ANSI"=w663:string[], "LT.Data.Languages.Unicode"=w661:string[], "LT.Data.Startup Language"=w657:string)
          n296 = local read "ListOfTextTranslations"() -> (w654:i32)
          n297 = local read "ListOfControls"() -> (w655:i32)
          n298 = property on="ListOfControls" class="MCListbox (strict)"("Val(Sgnl)"=w655) -> ()  [unwired: 2 in, 2 out]
          n299 = property on="ListOfTextTranslations" class="LstBox (strict)"("Val(Sgnl)"=w654) -> ()  [unwired: 2 in, 2 out]
          n300 = Build Array (concatenate)(w663, w661) -> (w658:string[])
          n301 = property on="DefLang" class="CmbBox"("Strings[]"=w663, "Value"=w656) -> ()  [unwired: 2 in, 2 out]
          n302 = property on="StartLang" class="CmbBox"("Strings[]"=w658, "Value"=w657) -> ()  [unwired: 2 in, 2 out]
          n303 = property on="Languages" class="LstBox (strict)"("Item Names"=w658) -> ()  [unwired: 2 in, 2 out]
        }
        frame "UI: VIs Update" {
          # "Stay in same selection"
          n304 = local read "App File Path"() -> (w664:path)
          n305 = Unbundle By Name(w670) -> ("LT.VIs"=w673:path[])
          n306 = for {
            tunnel: w673 -> [w681] mode=indexing
            tunnel: [w680] -> w674 mode=indexing
            n307 = Strip Path(path=w681) -> (name=w680:string)  [unwired: 1 out]
          }
          n308 = call "Get VI library name.vi"("App File Path"=w664, "VIs"=w673) -> ("Library or Error String"=w672:string[])  [unwired: 8 in, 1 out]
          n309 = property on="VIs" class="MCListbox (strict)"() -> ("ItemNames"=w677:string[][], "Value"=w676:i32)  [unwired: 2 in, 2 out]
          n310 = Build Array(w674, w672) -> (w675:string[][])
          n311 = Transpose 2D Array(2D array=w675) -> (transposed array=w669:string[][])
          n312 = Index Array(array=w669, index (col)=0 ("disabled index (col)")) -> (element=w667:string[])  [unwired: 1 in]
          n313 = Index Array(array=w677, index (row)=w676, index (col)=0 ("disabled index (col)")) -> (element=w666:string)
          n314 = Search 1D Array(1D array=w667, element=w666) -> (index of element=w665:i32)  [unwired: 1 in]
          n315 = property on="VIs" class="MCListbox (strict)"("ItemNames"=w669, "Value"=w665) -> ()  [unwired: 2 in, 2 out]
        }
        frame "UI: List Of Controls Update" {
          n316 = Unbundle By Name(w685) -> ("FP.Tr"=w683:map{string, T14}, "CTRLs"=w682:map{path, T17[]})
          n317 = call "Map to List of Ctrl.vi"("CTRLs"=w682, "FP.Tr"=w683) -> ("List of Ctrl"=w684:string[][])  [unwired: 9 in]
          n318 = property on="ListOfControls" class="MCListbox (strict)"("ItemNames"=w684) -> ()  [unwired: 2 in, 2 out]
        }
        frame "UI: VIs Update Controls" {
          # "Get curren selected controls."
          n319 = Unbundle By Name(w709) -> ("LT.Data.Languages.ANSI"=w704:string[], "LT.Data.Languages.Unicode"=w703:string[], "FP.Tr"=w694:map{string, T14}, "CTRLs"=w707:map{path, T17[]}, "LT.VIs"=w708:path[])
          n320 = property on="Controls" class="MCListbox (strict)"() -> ("ItemNames"=w693:string[][], "Value"=w688:i32[])  [unwired: 2 in, 2 out]
          n321 = Index Array(array=w693, index (col)=0 ("disabled index (col)")) -> (element=w689:string[])  [unwired: 1 in]
          n322 = for {
            tunnel: w689 -> [w713]
            tunnel: [w712] -> w690 mode=indexing
            tunnel: w688 -> [w711] mode=indexing
            n323 = Index Array(array=w713, index=w711) -> (element=w712:string)
          }
          n324 = Index Array(array=w708, index="VIs") -> (element=w706:path)
          n325 = Build Array (concatenate)(w704, w703) -> (w702:string[])
          n326 = Array Size(array=w702) -> (size(s)=w701:i32)
          n327 = call "VIs Filter Controls.vi"("ControlsFilter"="ControlsFilter", "VIs"=w707, "Path"=w706) -> ("Filtered Ctrls"=w705:T17[])  [unwired: 8 in]
          n328 = Unbundle By Name("ControlsFilter") -> ("NonTranslated"=w698:bool)
          n329 = for {
            tunnel: w705 -> [w732] mode=indexing
            tunnel: [w729] -> w696 mode=indexing if=w724
            tunnel: w701 -> [w728]
            tunnel: [w727] -> w695 mode=indexing if=w724
            tunnel: w698 -> [w723]
            tunnel: w694 -> [w722]
            tunnel: w690 -> [w718]
            tunnel: [w716] -> w691 mode=indexing if=w714
            i -> [w716]
            w726 = u16 38 items=["Untranslated"=37, "Translated"=38, "Some translated"=40] ("Item Symbol")
            # "Was the label selected?"
            n330 = Unbundle By Name(w732) -> ("Label"=w717:string, "Class Name"=w731:string, "Type"=w730:string)
            n331 = Look In Map(map=w722, key=w717) -> (key not found?=w719:bool, value=w721:T14)  [unwired: 1 in]
            n332 = Search 1D Array(1D array=w718, element=w717) -> (index of element=w715:i32)  [unwired: 1 in]
            n333 = Unbundle By Name(w721) -> ("Properties"=w720:T8[])
            n334 = Greater Or Equal To 0?(x=w715) -> (x >= 0?=w714:bool)
            n335 = call "Get Translations status symbol.vi"("Property"=w720, "Not found"=w719, "Number Of Languages"=w728) -> ("Item Symbol"=w727:i32, "State"=w733:string)  [unwired: 7 in]
            n336 = Build Array(w717, w731, w730, w733) -> (w729:string[])
            n337 = Not Equal?(x=w727, y=w726) -> (x != y?=w725:bool)
            n338 = Compound Arithmetic op=OR(w725, invert w723) -> (w724:bool)
          }
          n339 = property on="Controls" class="MCListbox (strict)"("ItemSyms"=w695, "ItemNames"=w696, "Val(Sgnl)"=w691) -> ()  [unwired: 2 in, 2 out]
        }
        frame "UI: FP Translation Filter ListOfControls" {
          # "Stay by last selection."
          n340 = local read "Search Label"() -> (w738:string)
          n341 = Unbundle By Name(w737) -> ("FP.Tr"=w735:map{string, T14}, "CTRLs"=w734:map{path, T17[]})
          n342 = call "Map to List of Ctrl.vi"("CTRLs"=w734, "FP.Tr"=w735) -> ("List of Ctrl"=w736:string[][])  [unwired: 9 in]
          n343 = To Lower Case(string=w738) -> (all lower case string=w740:string)
          n344 = Empty String/Path?(string/path=w740) -> (empty?=w749:bool)
          n345 = for {
            tunnel: w736 -> [w752] mode=indexing
            tunnel: [w762] -> w745 mode=indexing if=w760
            tunnel: w740 -> [w761]
            tunnel: w749 -> [w756]
            n346 = Index Array(array=w752, index=2) -> (element=w753:string)
            n347 = To Lower Case(string=w753) -> (all lower case string=w754:string)
            n348 = Match Pattern(string=w754, regular expression=w761) -> (offset past match=w759:i32)  [unwired: 1 in, 3 out]
            n349 = Greater Or Equal To 0?(x=w759) -> (x >= 0?=w758:bool)
            n350 = Or(x=w758, y=w756) -> (x .or. y?=w757:bool)
            n351 = case shown="True" w757 {
              tunnel: [_ w763] -> w762
              tunnel: [_ TRUE] -> w760
              tunnel: w752 -> [_ w763]
              frame False {
              }
              frame True {
              }
            }
          }
          n352 = property on="ListOfControls" class="MCListbox (strict)"() -> ("ItemNames"=w748:string[][], "Value"=w747:i32)  [unwired: 2 in, 2 out]
          n353 = Index Array(array=w748, index (row)=w747, index (col)=0 ("disabled index (col)")) -> (element=w742:string)
          n354 = Index Array(array=w745, index (col)=0 ("disabled index (col)")) -> (element=w743:string[])  [unwired: 1 in]
          n355 = Search 1D Array(1D array=w743, element=w742) -> (index of element=w741:i32)  [unwired: 1 in]
          n356 = property on="ListOfControls" class="MCListbox (strict)"("ItemNames"=w745, "Value"=w741, "TopLeft"=T11 {"Row"=0, "Column"=0} ("Top Left Visible Cell")) -> ()  [unwired: 2 in, 2 out]
        }
        frame "UI: FP Translation Show Translations" {
          # "Es wird über einen eigenen Case versucht nach dem Wechsel den gleichen Eintrag zu markieren!"
          # "The VI can be have some controls with same label name.\nDelete double entries."
          n357 = Unbundle By Name(w781) -> ("LT.Data"=w768:T16, "FP.Tr"=w767:map{string, T14}, "CTRLs"=w780:map{path, T17[]})
          n358 = local write "Label"(w770) -> ()
          n359 = invoke on="Tree" class="Tree (strict)" method="Edit Tree Items.Delete"(error in=w784, "Delete Children"=TRUE ("Delete Children?")) -> (error out=w783:errorcluster)  [unwired: 3 in, 4 out]
          n360 = for {
            tunnel: w780 -> [w795] mode=indexing
            tunnel: [w794] -> w769 mode=concatenating
            n361 = Unbundle By Name(w795) -> ("Ctrls"=w794:T17[])
          }
          n362 = call "Get Tree Items.vi"("Control.Label"=w770, "VIs.Ctrls"=w769, "FP.Tr"=w767, "Data"=w768) -> ("Used CTRL"=→"IsCtrlUsed":bool, "Caption.Visible"=→"Caption Unvisible":bool, "Selected CTRLs"=w772:T17[], "Use in VIs"=w766:string[], "Tree Items"=w786:T21, "Class Name"=→"Class Name":T3, "Comment"=w771:string)  [unwired: 1 in]
          n363 = local write "FP Translation Comment"(w771) -> ()
          n364 = invoke on="Tree" class="Tree (strict)" method="Edit Tree Items.Add Multiple Items to End"(error in=w783, "Items"=w786) -> (error out=w782:errorcluster)  [unwired: 2 in, 3 out]
          n365 = call "Remove Duplicates From 1D Array.vim"("array"=w766) -> ("array with duplicates removed"=w765:string[])  [unwired: 10 in]
          n366 = property on="VIs with Ctrl" class="LstBox (strict)"("Item Names"=w765) -> ()  [unwired: 2 in, 2 out]
          n367 = Array Size(array=w772) -> (size(s)=w774:i32)
          n368 = Decrement(x=w774) -> (x-1=w773:i32)
          n369 = disable-structure shown="Disabled" {
            frame Disabled {
              w787 = "" ("Tree")
              n370 = local write "Tree"(w787) -> ()
              n371 = local write "FPT.TextUnicode"(w787) -> ()
              n372 = local write "FPT.TextANSI"(w787) -> ()
            }
            frame Enabled {
            }
          }
          n373 = case shown="-1, 0" w773 {
            selector: w773 -> [_ w791]
            frame -1, 0 {
              n374 = property on="CTRL Index" class="DigNum (strict)"("Value"=0 ("CTRL Index"), "DisabledEnum"=T4."Disabled and Grayed Out" ("Disabled")) -> ()  [unwired: 2 in, 2 out]
            }
            frame Default {
              n375 = property on="CTRL Index" class="DigNum (strict)"("Increment"=1.0 ("Data Entry Limits:Increment"), "Maximum"=w791, "Minimum"=0.0 ("Data Entry Limits:Minimum"), "DisabledEnum"=T4."Enabled" ("Disabled")) -> ()  [unwired: 2 in, 2 out]
            }
          }
          n376 = Bundle By Name(cluster=w781, "Selected CTRLs"=w772) -> (w776:T18)
        }
        frame "UI: FP Translation Update Text Translations" {
          n377 = Match Pattern(string=w798, regular expression="_") -> (before substring=w797:string, match substring=w801:string, after substring=w800:string)  [unwired: 1 in, 1 out]
          n378 = case shown="Default" w801 {
            tunnel: w800 -> [_ w817]
            tunnel: w798 -> [_ w816]
            tunnel: w797 -> [_ w808]
            tunnel: [_ w807] -> w796
            frame "" {
            }
            frame Default {
              # "Set cursor to end of the text."
              n379 = call "Is Unicode.vi"("Language"=w817) -> ("Is Unicode"=w814:bool)
              n380 = property on="Tree" class="Tree (strict)"("Active Item Tag"=w816, "ActiveColNum"=1 ("Active Cell:Active Column Number")) -> ("Cell String"=w811:string)  [unwired: 2 in, 2 out]
              n381 = case shown="True" w814 {
                tunnel: [w818 w822] -> w813
                tunnel: w811 -> [w819 w826]
                tunnel: w808 -> [_ w827]
                tunnel: [_ w823] -> w807
                tunnel: [w818 w821] -> w806
                tunnel: [_ w820] -> w805
                frame False {
                  w818 = FALSE
                  n382 = local write "FPT.TextANSI"(w819) -> ()
                }
                frame True {
                  n383 = case shown="Default" w827 {
                    tunnel: w826 -> [w829 _]
                    tunnel: [w829 _] -> w824
                    tunnel: [_ w832] -> w823
                    tunnel: [w828 TRUE] -> w822
                    tunnel: [w828 _] -> w821
                    tunnel: [_ TRUE] -> w820
                    frame Default {
                      w828 = TRUE
                    }
                    frame "Plot Names" {
                      w832 = "The  language is not supported for the Plot Names!"  # Warninig
                    }
                  }
                  n384 = call "Delete Unicode Header.vi"("String in"=w824) -> ("String out"=w825:string)
                  n385 = local write "FPT.TextUnicode"(w825) -> ()
                }
              }
              n386 = String Length(string=w811) -> (length=w810:i32)
              n387 = Bundle(w810, w810) -> (w809:cluster{i32, i32})  [unwired: 1 in]
              n388 = Not(x=w813) -> (.not. x?=w812:bool)
              n389 = property on="FPT.TextUnicode" class="Str"("Visible"=w813, "Key Focus"=w806, "Text.Selection"=w809) -> ()  [unwired: 2 in, 2 out]
              n390 = property on="FPT.TextANSI" class="Str"("Visible"=w812, "Key Focus"=w812, "Text.Selection"=w809) -> ()  [unwired: 2 in, 2 out]
              n391 = property on="Warning" class="Str"("Visible"=w805) -> ()  [unwired: 2 in, 2 out]
            }
          }
          "Warning" <- w796
        }
        frame "UI: FP Translation Update ListOfVIs" {
          n392 = Match Pattern(string=w833, regular expression="_") -> (match substring=w836:string, after substring=w835:string)  [unwired: 1 in, 2 out]
          n393 = case shown="Default" w836 {
            tunnel: w835 -> [_ w848]
            tunnel: w833 -> [_ w847]
            frame "" {
            }
            frame Default {
              # "Set cursor to end of the text."
              n394 = call "Is Unicode.vi"("Language"=w848) -> ("Is Unicode"=w845:bool)
              n395 = property on="Tree" class="Tree (strict)"("Active Item Tag"=w847, "ActiveColNum"=1 ("Active Cell:Active Column Number")) -> ("Cell String"=w842:string)  [unwired: 2 in, 2 out]
              n396 = case shown="True" w845 {
                tunnel: [FALSE TRUE] -> w844
                tunnel: w842 -> [w850 w852]
                frame False {
                  n397 = local write "FPT.TextANSI"(w850) -> ()
                }
                frame True {
                  n398 = call "Delete Unicode Header.vi"("String in"=w852) -> ("String out"=w851:string)
                  n399 = local write "FPT.TextUnicode"(w851) -> ()
                }
              }
              n400 = String Length(string=w842) -> (length=w841:i32)
              n401 = Bundle(w841, w841) -> (w840:cluster{i32, i32})  [unwired: 1 in]
              n402 = Not(x=w844) -> (.not. x?=w843:bool)
              n403 = property on="FPT.TextUnicode" class="Str"("Visible"=w844, "Key Focus"=w844, "Text.Selection"=w840) -> ()  [unwired: 2 in, 2 out]
              n404 = property on="FPT.TextANSI" class="Str"("Visible"=w843, "Key Focus"=w843, "Text.Selection"=w840) -> ()  [unwired: 2 in, 2 out]
            }
          }
        }
        frame "UI: FP Translation Deactivate Controls" {
          n405 = local read "ListOfControls"() -> (w856:i32)
          n406 = case shown="Default" w856 {
            tunnel: [_ TRUE] -> w855
            tunnel: [T4."Disabled and Grayed Out" ("Disabled") T4."Enabled" ("Disabled")] -> w854
            frame -1 {
            }
            frame Default {
            }
          }
          n407 = property on="Caption Unvisible" class="Bool (strict)"("Visible"=w855) -> ()  [unwired: 2 in, 2 out]
          n408 = property on="IsCtrlUsed" class="Bool (strict)"("Visible"=w855) -> ()  [unwired: 2 in, 2 out]
          n409 = property on="DelCtrlToTranslate" class="Bool"("DisabledEnum"=w854) -> ()  [unwired: 2 in, 2 out]
        }
        frame "UI: FP Translation Update The Value ListOfVIs" {
          n410 = Unbundle By Name(w869) -> ("OldVal.ListOfVIs"=w867:string)
          n411 = property on="VIs with Ctrl" class="LstBox (strict)"() -> ("Item Names"=w868:string[])  [unwired: 2 in, 2 out]
          n412 = Search 1D Array(1D array=w868, element=w867) -> (index of element=w863:i32)  [unwired: 1 in]
          n413 = Less Than 0?(x=w863) -> (x < 0?=w866:bool)
          n414 = Select(t=0, s=w866, f=w863) -> (s? t:f=w865:i32)
          n415 = property on="VIs with Ctrl" class="LstBox (strict)"("Val(Sgnl)"=w865) -> ()  [unwired: 2 in, 2 out]
        }
        frame "UI: FP Translation Show Control" {
          n416 = Unbundle By Name(w885) -> ("Selected CTRLs"=w874:T17[])
          n417 = property on="VIs with Ctrl" class="LstBox (strict)"() -> ("Item Names"=w882:string[], "Value"=w881:i32)  [unwired: 2 in, 2 out]
          n418 = Index Array(array=w882, index=w881) -> (element=w880:string)
          n419 = call "Create VI Overview Picture.vi"("VI Name"=w880, "Selected CTRLs"=w874) -> ("image size"=w876:T12, "Origin"=w873:T10, "2D Picture"=→"2D Picture":picture)  [unwired: 7 in]
          n420 = for {
            N: 2 -> [_]
            tunnel: w876 -> [w901]
            tunnel: [w900] -> w875
            tunnel: w873 -> [w886]
            stop <- w887 stop-if-true
            # "Vertiical scroll was activated. Resize again."
            # "Activate the vertical scrollbar if \nthe max high is exeeded"
            n421 = property on="2D Picture" class="Pict"() -> ("Draw Area Size"=w903:T12, "VertScroll"=w888:bool)  [unwired: 2 in, 2 out]
            n422 = Divide(x=w903, y=w901) -> (x/y=w904:cluster{"Width":dbl, "Height":dbl})
            n423 = Unbundle By Name(w901) -> ("Height"=w895:u32)
            n424 = Unbundle By Name(w904) -> ("Width"=w900:dbl)
            n425 = Multiply(x=w900, y=w895) -> (x*y=w892:dbl)
            n426 = Not A Number/Path/Refnum?(number/path/refnum=w892) -> (NaN/Path/Refnum?=w893:bool)
            n427 = Select(t=u32 468 ("upper limit"), s=w893, f=w892) -> (s? t:f=w896:dbl)
            n428 = To Unsigned Long Integer(number=w896) -> (unsigned 32bit integer=w891:u32)
            n429 = In Range and Coerce(upper limit=u32 548, x=w891, lower limit=u32 0) -> (coerced(x)=w894:u32, In Range?=w890:bool)
            n430 = Bundle By Name(cluster=w903, "Height"=w894) -> (w902:T12)
            n431 = Not(x=w890) -> (.not. x?=w889:bool)
            n432 = property on="2D Picture" class="Pict"("ZoomFactor"=w900, "Origin"=w886, "Draw Area Size"=w902, "VertScroll"=w889) -> ()  [unwired: 2 in, 2 out]
            n433 = Implies(1:w888, 2:w889) -> (0:w887:bool)
          }
          n434 = local write "Button.ZoomToCtrl"(FALSE ("Button.ZoomToCtrl")) -> ()
          n435 = Bundle By Name(cluster=w885, "Origin"=w873, "ZoomOutFactor"=w875) -> (w878:T18)
        }
        frame "UI: FP Translation Zoom To CTRL" {
          w911 = i16 32767 ("upper limit")
          n436 = Unbundle By Name(w933) -> ("Selected CTRLs"=w931:T17[])
          n437 = Index Array(array=w931, index="CTRL Index") -> (element=w929:T17)
          n438 = Unbundle By Name(w929) -> ("refCtl"=w928:refnum<vi>, "refPane"=w905:refnum<vi>)
          n439 = call "Get CTRL Area.vi"("SizeOffset (16)"=u32 128 ("Offset (16)"), "error in (no error)"=w927, "Pane in"=w905, "Control in"=w928) -> ("error out"=w926:errorcluster, "CTRL Area"=w906:T22)  [unwired: 3 in, 3 out]
          n440 = Unbundle By Name(w906) -> ("right"=w925:i16, "left"=w910:i16, "bottom"=w919:i16, "top"=w914:i16)
          n441 = property on="2D Picture" class="Pict"() -> ("Draw Area Size"=w924:T12)  [unwired: 2 in, 2 out]
          n442 = Subtract(x=w925, y=w910) -> (x-y=w918:i16)
          n443 = Subtract(x=w919, y=w914) -> (x-y=w917:i16)
          n444 = Bundle(cluster=T12 {"Width"=0, "Height"=0} ("Draw Area Size"), "Width"=w918, "Height"=w917) -> (w916:T12)
          n445 = Divide(x=w924, y=w916) -> (x/y=w923:cluster{"Width":dbl, "Height":dbl})
          n446 = In Range and Coerce(upper limit=w911, x=w910, lower limit=i16 0) -> (coerced(x)=w909:i16)  [unwired: 1 out]
          n447 = In Range and Coerce(upper limit=w911, x=w914, lower limit=i16 0) -> (coerced(x)=w912:i16)  [unwired: 1 out]
          n448 = Unbundle By Name(w923) -> ("Width"=w922:dbl, "Height"=w921:dbl)
          n449 = Max & Min(x=w922, y=w921) -> (min(x,y)=w920:dbl)  [unwired: 1 out]
          n450 = property on="2D Picture" class="Pict"("ZoomFactor"=w920, "Left"=w909, "Top"=w912) -> ()  [unwired: 2 in, 2 out]
        }
        frame "UI: FP Translation Zoom Out" {
          n451 = Unbundle By Name(w936) -> ("ZoomOutFactor"=w935:dbl, "Origin"=w934:T10)
          n452 = property on="2D Picture" class="Pict"("ZoomFactor"=w935, "Origin"=w934) -> ()  [unwired: 2 in, 2 out]
        }
        frame "UI: FP Translation Update Control Visibility" {
          n453 = Unbundle By Name(w944) -> ("Selected CTRLs"=w942:T17[])
          n454 = Array Size(array=w942) -> (size(s)=w941:i32)
          n455 = case shown="Default" w941 {
            tunnel: [w948 w958] -> w946
            tunnel: [w947 w955] -> w940
            tunnel: w943 -> [w948 w954]
            tunnel: [w947 w950] -> w939
            tunnel: w942 -> [_ w949]
            frame 0 {
              w947 = TRUE ("InsideTheUI")
            }
            frame Default {
              n456 = local read "CTRL Index"() -> (w957:i32)
              n457 = Index Array(array=w949, index=w957) -> (element=w956:T17)
              n458 = Unbundle By Name(w956) -> ("refCtl"=w953:refnum<vi>, "refPane"=w951:refnum<vi>)
              n459 = call "Get CTRL Area.vi"("error in (no error)"=w954, "Pane in"=w951, "Control in"=w953) -> ("error out"=w959:errorcluster, "InsideTheUI"=w950:bool, "Control out"=w952:refnum<vi>)  [unwired: 4 in, 2 out]
              n460 = property class="Ctl"(reference=w952, error in=w959) -> (error out=w958:errorcluster, "Visible"=w955:bool)  [unwired: 1 out]
            }
          }
          "IsCtrlVisible" <- w940
          "IsCtrlInUIArea" <- w939
        }
        frame "---------- Macros ----------" {
          # "Macro: Macros have to be set in front of the states queue."
          # "Do not put any code in this frame.\n(It is a separator no-op. You can make a copy of this frame to create a new Macro frame)"
        }
        frame "Macro: Initialize" {
          # "Languages: Search initialisiert die Liste!"
          # "Macro: Macros have to be set in front of the states queue."
        }
        frame "Macro: Read Translation File" {
          # "Macro: Macros have to be set in front of the states queue."
        }
        frame "Macro: Import Translations" {
          # "Macro: Macros have to be set in front of the states queue."
          n461 = Format Into String(format string="Data: Init with Import >>%s\nData: Get VIs Controls\nUI: List Of Controls Update\nUI: File Changed", w971) -> (resulting string=w973:string)  [unwired: 2 in, 1 out]
        }
        frame "Macro: List Of Controls Value Change" {
          # "Macro: Macros have to be set in front of the states queue."
          n462 = local read "Tree"() -> (w983:string)
          n463 = call <vilib>:"Build State String with Arguments__JKI_lib_State_Machine.vi"("Arguments (\"\")"=w983, "State"="UI: FP Translation Update Text Translations") -> ("State with Arguments"=w984:string)  [unwired: 4 in]
          n464 = call <vilib>:"Build State String with Arguments__JKI_lib_State_Machine.vi"("Arguments (\"\")"=w977, "State"="UI: FP Translation Show Translations" ("State(s) at Back (\"\")")) -> ("State with Arguments"=w982:string)  [unwired: 4 in]
          n465 = call <vilib>:"Add State(s) to Queue__JKI_lib_State_Machine.vi"("State(s) in Front (\"\")"=w982, "State(s) in (\"\")"=w984, "State(s) at Back (\"\")"="UI: FP Translation Deactivate Controls\nUI: FP Translation Update The Value ListOfVIs" ("State(s) at Back (\"\")")) -> ("States Out"=w978:string)  [unwired: 12 in]
        }
        frame "Macro: Release" {
          # "Do not edit\n\nJune 16, 2025 - The \"Data Save\" feature had to be removed,\notherwise changes would have been saved without the user's consent!"
          # "Macro: Macros have to be set in front of the states queue."
          n466 = Unbundle By Name(w993) -> ("Core.Close Panel on Exit?"=w995:bool)
          n467 = Select(t="UI: Set FP State >> Close", s=w995, f="") -> (s? t:f=w990:string)
          n468 = call <vilib>:"Add State(s) to Queue__JKI_lib_State_Machine.vi"("State(s) in (\"\")"=w990, "State(s) at Back (\"\")"="Data: Update Config\n//Data: Save\nData: Cleanup") -> ("States Out"=w992:string)  [unwired: 13 in]
        }
        frame "---------- General ----------" {
          # "Modul Separator\n(You can make a copy of, or modify, this frame)"
        }
        frame "General: File Save As" {
          n469 = local read "Language Config Path"() -> (w1000:path)
          n470 = call "File Dialog"("pattern (all files)"="*.json") -> ("selected path"=w1004:path, "cancelled"=w1005:bool)  [unwired: 11 in, 2 out]
          n471 = case shown="False" w1005 {
            tunnel: w1002 -> [w1012 w1013]
            tunnel: [w1011 w1013] -> w1001
            tunnel: w1004 -> [w1010 _]
            tunnel: w1000 -> [w1008 _]
            frame False {
              n472 = Copy(8:w1012, 9:TRUE ("overwrite (F)"), 10:w1010, 11:w1008) -> (0:w1011:errorcluster)  [unwired: 1 in, 2 out]
            }
            frame True {
            }
          }
        }
        frame "General: Export to txt" {
          n473 = local read "Language Config Path"() -> (w1023:path)
          n474 = Unbundle By Name(w1027) -> ("LT.Data.Languages"=w1024:cluster{"ANSI":string[], "Unicode":string[]}, "LT.FP Translations"=w1026:T7[], "LT.Text Translations"=w1019:T7[])
          n475 = call "File Dialog4"() -> ("selected path"=w1021:path, "cancelled"=w1014:bool, "error out"=w1015:errorcluster)  [unwired: 12 in, 1 out]
          n476 = Build Array(w1026, w1019) -> (w1020:T7[][])
          n477 = call <vilib>:"Get File Extension.vi"("error in (no error)"=w1016, "file"=w1023) -> ("error out"=w1017:errorcluster, "filename without extension"=w1022:string)  [unwired: 5 in, 3 out]
          n478 = case shown="False" w1014 {
            tunnel: [w1035 w1062] -> w1025
            tunnel: w1024 -> [w1034 _]
            tunnel: w1022 -> [w1033 _]
            tunnel: w1021 -> [w1032 _]
            tunnel: w1020 -> [w1031 _]
            tunnel: string[] ["Frontpanel", "Text"] ("input 1") -> [w1030 _]
            tunnel: w1017 -> [w1029 w1062]
            tunnel: w1015 -> [_ _]
            frame False {
              n479 = for {
                tunnel: w1031 -> [w1038] mode=indexing
                tunnel: w1034 -> [w1039]
                tunnel: w1033 -> [w1043]
                tunnel: w1032 -> [w1045]
                shift-right: [w1048] -> w1035
                shift-left: w1029 -> [w1049]
                tunnel: w1030 -> [w1042] mode=indexing
                w1050 = T23."replace or create" ("operation (0:open)")
                n480 = call "Format Data for ANSI-Export.vi"("LT.Data.Languages"=w1039, "Translations"=w1038) -> ("ANSI string"=w1057:string)  [unwired: 9 in]
                n481 = Format Into String(format string="%s_%s_ansi.txt", w1043, w1042) -> (resulting string=w1054:string)  [unwired: 2 in, 1 out]
                n482 = Format Into String(format string="%s_%s_unicode.txt", w1043, w1042) -> (resulting string=w1046:string)  [unwired: 2 in, 1 out]
                n483 = call "Format Data for Unicode-Export.vi"("LT.Data.Languages"=w1039, "Translations"=w1038) -> ("string"=w1037:string)  [unwired: 9 in]
                n484 = Build Path(base path=w1045, name or relative path=w1054) -> (appended path=w1053:path)
                n485 = Build Path(base path=w1045, name or relative path=w1046) -> (appended path=w1041:path)
                n486 = Open/Create/Replace File(file path (use dialog)=w1053, error in=w1049, operation (0:open)=w1050) -> (refnum out=w1061:refnum<file>, error out=w1059:errorcluster)  [unwired: 3 in, 1 out]
                n487 = Open/Create/Replace File(file path (use dialog)=w1041, error in=w1049, operation (0:open)=w1050) -> (refnum out=w1036:refnum<file>, error out=w1051:errorcluster)  [unwired: 3 in, 1 out]
                n488 = Write to Text File(file (use dialog)=w1061, text=w1057, error in=w1059) -> (refnum out=w1060:refnum<file>, error out=w1058:errorcluster)  [unwired: 1 in, 1 out]
                n489 = Write to Text File(file (use dialog)=w1036, text=w1037, error in=w1051) -> (refnum out=w1040:refnum<file>, error out=w1052:errorcluster)  [unwired: 1 in, 1 out]
                n490 = Close File(refnum=w1060, error in=w1058) -> (error out=w1056:errorcluster)  [unwired: 1 out]
                n491 = Close File(refnum=w1040, error in=w1052) -> (error out=w1047:errorcluster)  [unwired: 1 out]
                n492 = Merge Errors(w1056, w1047) -> (w1048:errorcluster)
              }
            }
            frame True {
            }
          }
        }
        frame "---------- Languages ----------" {
        }
        frame "Languages: Add" {
          # "#ToDo\nInsert Sound if the language allready exist."
          n493 = in-place {
            n494 = in-place-cluster #4(w1068) -> ("LT.Data.Languages.Unicode"=w1080:string[], "LT.Data.Languages.ANSI"=w1079:string[], "FP.Tr"=w1078:map{string, T14}, "T.Tr"=w1077:map{string, T14})
            n495 = property on="AllLanguages" class="LstBox (strict)"() -> ("Item Names"=w1072:string[], "Value"=w1071:i32)  [unwired: 2 in, 2 out]
            n496 = Index Array(array=w1072, index=w1071) -> (element=w1070:string)
            n497 = call "Is Unicode.vi"("Language"=w1070) -> ("Is Unicode"=w1081:bool)
            n498 = case shown="True" w1081 {
              tunnel: w1079 -> [w1088 w1110]
              tunnel: [w1089 w1110] -> w1075
              tunnel: w1080 -> [w1087 w1113]
              tunnel: [w1087 w1109] -> w1076
              tunnel: w1078 -> [w1086 w1108]
              tunnel: w1077 -> [w1083 w1106]
              tunnel: [w1084 w1105] -> w1073
              tunnel: [w1085 w1107] -> w1074
              tunnel: w1070 -> [w1082 w1104]
              frame False {
                # "ANSI language"
                n499 = Search 1D Array(1D array=w1088, element=w1082) -> (index of element=w1091:i32)  [unwired: 1 in]
                n500 = Less Than 0?(x=w1091) -> (x < 0?=w1090:bool)
                n501 = case shown="False" w1090 {
                  tunnel: w1088 -> [w1095 w1099]
                  tunnel: w1082 -> [_ w1096]
                  tunnel: [w1095 w1098] -> w1089
                  tunnel: w1086 -> [w1094 w1103]
                  tunnel: [w1094 w1102] -> w1085
                  tunnel: [w1093 w1100] -> w1084
                  tunnel: w1083 -> [w1093 w1101]
                  frame False {
                    n502 = call <vilib>:"Beep.vi"("use system alert? (T)"=TRUE) -> ()  [unwired: 11 in]
                  }
                  frame True {
                    w1097 = TRUE
                    n503 = Build Array (concatenate)(w1099, w1096) -> (w1098:string[])
                    n504 = call "Add Language to Controls.vi"("ANSI"=w1097, "Translastions in"=w1103) -> ("Translastions out"=w1102:map{string, T14})  [unwired: 9 in]
                    n505 = call "Add Language to Controls.vi"("ANSI"=w1097, "Translastions in"=w1101) -> ("Translastions out"=w1100:map{string, T14})  [unwired: 9 in]
                  }
                }
              }
              frame True {
                # "Unicode language"
                n506 = Search 1D Array(1D array=w1113, element=w1104) -> (index of element=w1112:i32)  [unwired: 1 in]
                n507 = Less Than 0?(x=w1112) -> (x < 0?=w1111:bool)
                n508 = case shown="True" w1111 {
                  tunnel: w1113 -> [w1117 w1119]
                  tunnel: [w1117 w1124] -> w1109
                  tunnel: w1104 -> [_ w1125]
                  tunnel: w1108 -> [w1116 w1123]
                  tunnel: [w1116 w1122] -> w1107
                  tunnel: w1106 -> [w1115 w1121]
                  tunnel: [w1115 w1120] -> w1105
                  frame False {
                    n509 = call <vilib>:"Beep.vi"("use system alert? (T)"=TRUE) -> ()  [unwired: 11 in]
                  }
                  frame True {
                    w1118 = FALSE ("ANSI")
                    n510 = call "Add Language to Controls.vi"("ANSI"=w1118, "Translastions in"=w1123) -> ("Translastions out"=w1122:map{string, T14})  [unwired: 9 in]
                    n511 = Build Array (concatenate)(w1119, w1125) -> (w1124:string[])
                    n512 = call "Add Language to Controls.vi"("ANSI"=w1118, "Translastions in"=w1121) -> ("Translastions out"=w1120:map{string, T14})  [unwired: 9 in]
                  }
                }
              }
            }
            n513 = in-place-cluster #4("LT.Data.Languages.Unicode"=w1076, "LT.Data.Languages.ANSI"=w1075, "FP.Tr"=w1074, "T.Tr"=w1073) -> (w1067:T18)
          }
        }
        frame "Languages: Delete" {
          n514 = in-place {
            w1132 = 1 ("length")
            n515 = in-place-cluster #5(w1128) -> ("LT.Data.Languages.ANSI"=w1137:string[], "LT.Data.Languages.Unicode"=w1135:string[], "FP.Tr"=w1143:map{string, T14}, "T.Tr"=w1141:map{string, T14})
            n516 = property on="Languages" class="LstBox (strict)"() -> ("Item Names"=w1138:string[], "Value"=w1139:i32)  [unwired: 2 in, 2 out]
            n517 = Index Array(array=w1138, index=w1139) -> (element=w1134:string)
            n518 = Search 1D Array(1D array=w1137, element=w1134) -> (index of element=w1130:i32)  [unwired: 1 in]
            n519 = Search 1D Array(1D array=w1135, element=w1134) -> (index of element=w1131:i32)  [unwired: 1 in]
            n520 = Delete From Array(array=w1137, length=w1132, index=w1130) -> (array with subset deleted=w1136:string[])  [unwired: 1 out]
            n521 = Delete From Array(array=w1135, length=w1132, index=w1131) -> (array with subset deleted=w1133:string[])  [unwired: 1 out]
            n522 = call "Remove Language from translations.vi"("Unicode Index"=w1131, "ANSI Index"=w1130, "Translastions in"=w1143) -> ("Translastions out"=w1142:map{string, T14})  [unwired: 8 in]
            n523 = call "Remove Language from translations.vi"("Unicode Index"=w1131, "ANSI Index"=w1130, "Translastions in"=w1141) -> ("Translastions out"=w1140:map{string, T14})  [unwired: 8 in]
            n524 = in-place-cluster #5("LT.Data.Languages.ANSI"=w1136, "LT.Data.Languages.Unicode"=w1133, "FP.Tr"=w1142, "T.Tr"=w1140) -> (w1127:T18)
          }
        }
        frame "Languages: Search" {
          n525 = call-poly <vilib>:"Convert UTF-16LE to ASCII.vi"("Unicode"="E\u0000n\u0000g\u0000l\u0000i\u0000s\u0000h\u0000,\u0000 \u0000S\u0000p\u0000a\u0000n\u0000i\u0000s\u0000h\u0000,\u0000 \u0000P\u0000o\u0000r\u0000t\u0000u\u0000g\u0000u\u0000e\u0000s\u0000e\u0000,\u0000 \u0000F\u0000r\u0000e\u0000n\u0000c\u0000h\u0000,\u0000 \u0000G\u0000e\u0000r\u0000m\u0000a\u0000n\u0000,\u0000 \u0000I\u0000t\u0000a\u0000l\u0000i\u0000a\u0000n\u0000,\u0000 \u0000D\u0000u\u0000t\u0000c\u0000h\u0000,\u0000 \u0000R\u0000u\u0000s\u0000s\u0000i\u0000a\u0000n\u0000,\u0000 \u0000C\u0000h\u0000i\u0000n\u0000e\u0000s\u0000e\u0000,\u0000 \u0000A\u0000r\u0000a\u0000b\u0000i\u0000c\u0000,\u0000 \u0000A\u0000l\u0000b\u0000a\u0000n\u0000i\u0000a\u0000n\u0000,\u0000 \u0000A\u0000r\u0000m\u0000e\u0000n\u0000i\u0000a\u0000n\u0000,\u0000 \u0000B\u0000e\u0000n\u0000g\u0000a\u0000l\u0000i\u0000,\u0000 \u0000B\u0000o\u0000s\u0000n\u0000i\u0000a\u0000n\u0000,\u0000 \u0000B\u0000u\u0000l\u0000g\u0000a\u0000r\u0000i\u0000a\u0000n\u0000,\u0000 \u0000C\u0000a\u0000t\u0000a\u0000l\u0000a\u0000n\u0000,\u0000 \u0000C\u0000r\u0000o\u0000a\u0000t\u0000i\u0000a\u0000n\u0000,\u0000 \u0000C\u0000z\u0000e\u0000c\u0000h\u0000,\u0000 \u0000D\u0000a\u0000n\u0000i\u0000s\u0000h\u0000,\u0000 \u0000F\u0000i\u0000n\u0000n\u0000i\u0000s\u0000h\u0000,\u0000 \u0000G\u0000a\u0000l\u0000i\u0000c\u0000i\u0000a\u0000n\u0000,\u0000 \u0000G\u0000r\u0000e\u0000e\u0000k\u0000,\u0000 \u0000H\u0000e\u0000b\u0000r\u0000e\u0000w\u0000,\u0000 \u0000H\u0000i\u0000n\u0000d\u0000i\u0000,\u0000 \u0000H\u0000u\u0000n\u0000g\u0000a\u0000r\u0000i\u0000a\u0000n\u0000,\u0000 \u0000J\u0000a\u0000p\u0000a\u0000n\u0000e\u0000s\u0000e\u0000,\u0000 \u0000K\u0000o\u0000r\u0000e\u0000a\u0000n\u0000,\u0000 \u0000P\u0000o\u0000l\u0000i\u0000s\u0000h\u0000,\u0000 \u0000P\u0000u\u0000n\u0000j\u0000a\u0000b\u0000i\u0000,\u0000 \u0000R\u0000o\u0000m\u0000a\u0000n\u0000i\u0000a\u0000n\u0000,\u0000 \u0000S\u0000e\u0000r\u0000b\u0000i\u0000a\u0000n\u0000,\u0000 \u0000S\u0000l\u0000o\u0000v\u0000a\u0000k\u0000,\u0000 \u0000S\u0000l\u0000o\u0000v\u0000e\u0000n\u0000e\u0000,\u0000 \u0000T\u0000u\u0000r\u0000k\u0000i\u0000s\u0000...") -> ("ASCII"=w1144:string)  [unwired: 4 in]
          n526 = local read "Search"() -> (w1149:string)
          n527 = call <vilib>:"Delimited String to 1D String Array.vi"("delimiter"=",", "delimited string"=w1144) -> ("string array"=w1148:string[])  [unwired: 9 in]
          n528 = To Upper Case(1:w1149) -> (0:w1151:string)
          n529 = for {
            tunnel: w1151 -> [w1158]
            tunnel: w1148 -> [w1157] mode=indexing
            tunnel: [w1155] -> w1152 mode=indexing if=w1156
            n530 = call <vilib>:"Trim Whitespace.vi"("string"=w1157) -> ("trimmed string"=w1155:string)  [unwired: 1 in]
            n531 = String Length(string=w1158) -> (length=w1161:i32)
            n532 = To Upper Case(1:w1155) -> (0:w1160:string)
            n533 = String Subset(string=w1160, length (rest)=w1161) -> (substring=w1159:string)  [unwired: 1 in]
            n534 = Equal?(x=w1159, y=w1158) -> (x = y?=w1156:bool)
          }
          n535 = property on="AllLanguages" class="LstBox (strict)"("Top Row"=0) -> ()  [unwired: 2 in, 2 out]
          n536 = property on="AllLanguages" class="LstBox (strict)"("Item Names"=w1152) -> ()  [unwired: 2 in, 2 out]
        }
        frame "---------- VIs ----------" {
        }
        frame "VIs: Add VI" {
          n537 = local read "App File Path"() -> (w1165:path)
          n538 = call "File Dialog3"("start path"=w1165, "prompt"="Select a VI", "pattern (all files)"="*.vi" ("pattern label"), "pattern label"="Virtual Instrument") -> ("selected path"=w1174:path, "cancelled"=w1176:bool, "error out"=w1179:errorcluster)  [unwired: 8 in, 1 out]
          n539 = Not(x=w1176) -> (.not. x?=w1177:bool)
          n540 = call <vilib>:"Is Path and Not Empty.vi"("path"=w1174) -> ("Is Path and Not Empty?"=w1175:bool)  [unwired: 4 in]
          n541 = call <vilib>:"Clear Errors.vi"("error in (no error)"=w1179) -> ()  [unwired: 5 in, 2 out]
          n542 = And(x=w1177, y=w1175) -> (x .and. y?=w1178:bool)
          n543 = case shown="True" w1178 {
            tunnel: w1170 -> [w1181 w1185]
            tunnel: [w1181 w1184] -> w1169
            tunnel: w1174 -> [_ w1187]
            tunnel: w1165 -> [_ w1186]
            tunnel: w1167 -> [w1180 w1183]
            tunnel: [w1180 w1182] -> w1166
            frame False {
            }
            frame True {
              n544 = in-place {
                in-place-border: w1187 -> [w1191]
                in-place-border: w1186 -> [w1197]
                in-place-border: w1183 -> [w1193]
                in-place-border: [w1192] -> w1182
                # "The files are the path relativ to the\napplications directory."
                n545 = in-place-cluster #6(w1185) -> ("LT.VIs"=w1190:path[], "CTRLs"=w1195:map{path, T17[]})
                n546 = call <vilib>:"Compare Two Paths.vi"("Path 2"=w1191, "Path 1"=w1197) -> ("Relative Path from 1 to 2"=w1189:path)  [unwired: 6 in, 3 out]
                n547 = Search 1D Array(1D array=w1190, element=w1189) -> (index of element=w1188:i32)  [unwired: 1 in]
                n548 = case shown="-1" w1188 {
                  tunnel: [w1200 w1209] -> w1196
                  tunnel: w1195 -> [w1199 w1208]
                  tunnel: [w1199 w1207] -> w1194
                  tunnel: w1193 -> [w1198 w1205]
                  tunnel: [w1198 w1204] -> w1192
                  tunnel: w1191 -> [_ w1203]
                  tunnel: w1190 -> [w1200 w1202]
                  tunnel: w1189 -> [_ w1201]
                  frame Default {
                    # "VI is already\nexixst."
                  }
                  frame -1 {
                    n549 = Build Array (concatenate)(w1202, w1201) -> (w1209:path[])
                    n550 = call "Get All Controls.vi"("error in (no error)"=w1205, "VI"=w1203) -> ("error out"=w1204:errorcluster, "VIs Controls"=w1206:T17[])  [unwired: 8 in]
                    n551 = Insert Into Map(map in=w1208, key=w1201, value=w1206) -> (map out=w1207:map{path, T17[]})  [unwired: 2 out]
                  }
                }
                n552 = in-place-cluster #6("LT.VIs"=w1196, "CTRLs"=w1194) -> (w1184:T18)
              }
            }
          }
        }
        frame "VIs: Delete VI" {
          n553 = in-place {
            n554 = in-place-cluster #7(w1211) -> ("CTRLs"=w1215:map{path, T17[]}, "LT.VIs"=w1219:path[])
            n555 = local read "VIs"() -> (w1217:i32)
            n556 = Decrement(x=w1217) -> (x-1=w1216:i32)
            n557 = Delete From Array(array=w1219, index=w1217) -> (deleted portion=w1220:path, array with subset deleted=w1218:path[])  [unwired: 1 in]
            n558 = property on="VIs" class="MCListbox (strict)"("Val(Sgnl)"=w1216) -> ()  [unwired: 2 in, 2 out]
            n559 = Remove From Map(10:w1220, 11:w1215) -> (3:w1214:map{path, T17[]})  [unwired: 2 out]
            n560 = in-place-cluster #7("CTRLs"=w1214, "LT.VIs"=w1218) -> (w1210:T18)
          }
        }
        frame "VIs: Sort" {
          n561 = in-place {
            n562 = in-place-cluster #8(w1222) -> ("LT.VIs"=w1226:path[])
            n563 = Sort 1D Array(array=w1226) -> (sorted array=w1225:path[])
            n564 = in-place-cluster #8("LT.VIs"=w1225) -> (w1221:T18)
          }
        }
        frame "VIs: Show Frontpanel" {
          n565 = Unbundle By Name(w1238) -> ("LT.VIs"=w1232:path[])
          n566 = local read "VIs"() -> (w1231:i32)
          n567 = local read "App File Path"() -> (w1227:path)
          n568 = Index Array(array=w1232, index=w1231) -> (element=w1236:path)
          n569 = Greater Or Equal To 0?(x=w1231) -> (x >= 0?=w1235:bool)
          n570 = call <vilib>:"Is Path and Not Empty.vi"("path"=w1236) -> ("Is Path and Not Empty?"=w1233:bool)  [unwired: 4 in]
          n571 = And(x=w1233, y=w1235) -> (x .and. y?=w1234:bool)
          n572 = Build Path(base path=w1227, name or relative path=w1236) -> (appended path=w1237:path)
          n573 = case shown="True" w1234 {
            tunnel: w1237 -> [_ w1246]
            tunnel: w1230 -> [w1239 w1245]
            tunnel: [w1239 w1241] -> w1229
            frame False {
            }
            frame True {
              n574 = Open VI Reference(vi path=w1246, error in (no error)=w1245) -> (vi reference=w1244:refnum<vi>, error out=w1243:errorcluster)  [unwired: 4 in]
              n575 = invoke class="VI" method="FP.Open"(reference=w1244, error in=w1243) -> (reference out=w1240:refnum<vi>, error out=w1242:errorcluster)  [unwired: 3 in, 3 out]
              n576 = Close Reference(reference=w1240, error in (no error)=w1242) -> (error out=w1241:errorcluster)
            }
          }
        }
        frame "---------- FP Translation ----------" {
        }
        frame "FP Translation: Add Control" {
          n577 = in-place {
            in-place-border: w1251 -> [w1255]
            n578 = in-place-cluster #9(w1253) -> ("FP.Tr"=w1257:map{string, T14})
            n579 = in-place {
              n580 = in-place-map #10(w1257, w1255) -> ()  [unwired: 1 in, 2 out]
              n581 = in-place-map #10(T14 {"Tags"="", "Comment"="", "Properties"=[]} ("value"), LVMapReplaceAction."Add or Modify Entry" ("action")) -> (w1256:map{string, T14})  [unwired: 2 out]
            }
            n582 = in-place-cluster #9("FP.Tr"=w1256) -> (w1252:T18)
          }
        }
        frame "FP Translation: Delete Control" {
          n583 = in-place {
            w1271 = 0 ("disabled index (col)")
            n584 = in-place-cluster #11(w1261) -> ("FP.Tr"=w1270:map{string, T14})
            n585 = property on="ListOfControls" class="MCListbox (strict)"() -> ("ItemNames"=w1267:string[][], "Value"=w1265:i32)  [unwired: 2 in, 2 out]
            n586 = Delete From Array(array=w1267, length=1, index (row)=w1265) -> (deleted portion=w1272:string[][], array with subset deleted=w1266:string[][])  [unwired: 1 in]
            n587 = Decrement(x=w1265) -> (x-1=w1264:i32)
            n588 = Index Array(array=w1272, index (row)=w1271, index (col)=w1271) -> (element=w1273:string)
            n589 = property on="ListOfControls" class="MCListbox (strict)"("ItemNames"=w1266, "Val(Sgnl)"=w1264) -> ()  [unwired: 2 in, 2 out]
            n590 = Remove From Map(10:w1273, 11:w1270) -> (3:w1269:map{string, T14})  [unwired: 2 out]
            n591 = in-place-cluster #11("FP.Tr"=w1269) -> (w1260:T18)
          }
        }
        frame "FP Translation: Rename Control" {
          n592 = in-place {
            in-place-border: w1275 -> [w1287]
            # "Get old control name."
            n593 = in-place-cluster #12(w1277) -> ("FP.Tr"=w1283:map{string, T14})
            n594 = property on="ListOfControls" class="MCListbox (strict)"() -> ("ItemNames"=w1286:string[][], "Value"=w1284:i32)  [unwired: 2 in, 2 out]
            n595 = Index Array(array=w1286, index (row)=w1284, index (col)=0 ("disabled index (col)")) -> (element=w1279:string)
            n596 = Remove From Map(10:w1279, 11:w1283) -> (1:w1280:T14, 3:w1282:map{string, T14})  [unwired: 1 out]
            n597 = Insert Into Map(map in=w1282, key=w1287, value=w1280) -> (map out=w1281:map{string, T14})  [unwired: 2 out]
            n598 = in-place-cluster #12("FP.Tr"=w1281) -> (w1276:T18)
          }
        }
        frame "FP Translation: Edit Properties" {
          n599 = Unbundle By Name(w1289) -> ("LT.Data.Languages"=w1288:cluster{"ANSI":string[], "Unicode":string[]})
          n600 = in-place {
            in-place-border: w1288 -> [w1294]
            n601 = in-place-cluster #13(w1289) -> ("FP.Tr"=w1297:map{string, T14})
            n602 = local read "Tree"() -> (w1293:string)
            n603 = property on="Tree" class="Tree (strict)"("ActiveColNum"=1 ("Active Cell:Active Column Number"), "Active Item Tag"=w1293) -> ("Cell String"=w1298:string)  [unwired: 2 in, 2 out]
            n604 = local read "Label"() -> (w1295:string)
            n605 = call "Edit Property In Translation.vi"("Languages"=w1294, "Property_Language"=w1293, "Translations Text"=w1298, "Control Label Name"=w1295, "Translastions in"=w1297) -> ("Translastions out"=w1296:map{string, T14})  [unwired: 6 in]
            n606 = in-place-cluster #13("FP.Tr"=w1296) -> (w1291:T18)
          }
        }
        frame "FP Translation: Look for Next unused CTRL" {
          # "Get Tags"
          n607 = local read "ListOfControls"() -> (w1301:i32)
          n608 = property on="ListOfControls" class="MCListbox (strict)"() -> ("ItemNames"=w1300:string[][])  [unwired: 2 in, 2 out]
          n609 = Increment(x=w1301) -> (x+1=w1303:i32)
          n610 = Index Array(array=w1300, index (col)=2 ("disabled index (col)")) -> (element=w1308:string[])  [unwired: 1 in]
          n611 = Split 1D Array(array=w1308, index=w1303) -> (first subarray=w1309:string[], second subarray=w1314:string[])
          n612 = Array Size(array=w1308) -> (size(s)=w1307:i32)
          n613 = Array Size(array=w1309) -> (size(s)=w1304:i32)
          n614 = Build Array (concatenate)(w1314, w1309) -> (w1313:string[])
          n615 = for {
            tunnel: w1313 -> [w1324] mode=indexing
            tunnel: [w1320] -> w1312
            tunnel: [w1323] -> w1305
            i -> [w1323]
            stop <- w1320 stop-if-true
            n616 = To Lower Case(string=w1324) -> (all lower case string=w1322:string)
            n617 = Match Pattern(string=w1322, regular expression="unused") -> (offset past match=w1319:i32)  [unwired: 1 in, 3 out]
            n618 = Greater Or Equal To 0?(x=w1319) -> (x >= 0?=w1320:bool)
          }
          n619 = Add(x=w1304, y=w1305) -> (x+y=w1318:i32)
          n620 = Quotient & Remainder(x=w1318, y=w1307) -> (x-y*floor(x/y)=w1306:i32)  [unwired: 1 out]
          n621 = Select(t=w1306, s=w1312, f=-1 ("Value (Signaling)")) -> (s? t:f=w1311:i32)
          n622 = property on="ListOfControls" class="MCListbox (strict)"("Val(Sgnl)"=w1311) -> ()  [unwired: 2 in, 2 out]
        }
        frame "---------- Text Translation ----------" {
        }
        frame "Text Translation: Show Translation" {
          # "Falls kein Eintrag markiert war, min.\nden 0. Eintrag highlighten!"
          n623 = Unbundle By Name(w1349) -> ("LT.Data.Languages.ANSI"=w1340:string[], "LT.Data.Languages.Unicode"=w1339:string[], "T.Tr"=w1344:map{string, T14})
          n624 = property on="ListOfTextTranslations" class="LstBox (strict)"() -> ("Item Names"=w1348:string[], "Value"=w1347:i32)  [unwired: 2 in, 2 out]
          n625 = Index Array(array=w1348, index=w1347) -> (element=w1343:string)
          n626 = Look In Map(map=w1344, key=w1343) -> (value=w1342:T14)  [unwired: 1 in, 1 out]
          n627 = local write "TextName"(w1343) -> ()
          n628 = Build Array (concatenate)(w1340, w1339) -> (w1338:string[])
          n629 = Unbundle By Name(w1342) -> ("Properties"=w1341:T8[])
          n630 = Index Array(array=w1341) -> (element=w1346:T8)  [unwired: 1 in]
          n631 = Unbundle By Name(w1346) -> ("Translation ANSI"=w1345:string[], "Translation Unicode"=w1334:string[])
          n632 = local read "TextTranslation"() -> (w1331:i32)
          n633 = call "Add Unicode Header.vi"("Array"=w1334) -> ("Array with header 2"=w1333:string[])  [unwired: 1 in, 1 out]
          n634 = Build Array (concatenate)(w1345, w1333) -> (w1332:string[])
          n635 = In Range and Coerce(upper limit=123456789, x=w1331, lower limit=0) -> (coerced(x)=w1330:i32)  [unwired: 1 out]
          n636 = Build Array(w1338, w1332) -> (w1337:string[][])
          n637 = Transpose 2D Array(2D array=w1337) -> (transposed array=w1336:string[][])
          n638 = property on="TextTranslation" class="MCListbox (strict)"("ItemNames"=w1336, "Value"=w1330) -> ()  [unwired: 2 in, 2 out]
        }
        frame "Text Translation: Value Change" {
          n639 = property on="TextTranslation" class="MCListbox (strict)"() -> ("ItemNames"=w1355:string[][], "Value"=w1351:i32)  [unwired: 2 in, 2 out]
          n640 = Index Array(array=w1355, index (row) #1=w1351, index (col) #1=0 ("disabled index (col)"), index (row) #2=w1351, index (col) #2=1 ("disabled index (col)")) -> (element #1=w1356:string, element #2=w1359:string)
          n641 = call "Is Unicode.vi"("Language"=w1356) -> ("Is Unicode"=w1357:bool)
          n642 = case shown="True" w1357 {
            selector: w1357 -> [_ w1366]
            tunnel: w1359 -> [w1365 w1368]
            tunnel: [_ w1366] -> w1361
            frame False {
              n643 = local write "TT.TextANSI"(w1365) -> ()
            }
            frame True {
              n644 = call "Delete Unicode Header.vi"("String in"=w1368) -> ("String out"=w1367:string)
              n645 = local write "TT.TextUnicode"(w1367) -> ()
            }
          }
          n646 = String Length(string=w1359) -> (length=w1358:i32)
          n647 = Bundle(w1358, w1358) -> (w1354:cluster{i32, i32})  [unwired: 1 in]
          n648 = Not(x=w1361) -> (.not. x?=w1360:bool)
          n649 = property on="TT.TextUnicode" class="Str"("Visible"=w1361, "Key Focus"=w1361, "Text.Selection"=w1354) -> ()  [unwired: 2 in, 2 out]
          n650 = property on="TT.TextANSI" class="Str"("Visible"=w1360, "Key Focus"=w1360, "Text.Selection"=w1354) -> ()  [unwired: 2 in, 2 out]
        }
        frame "Text Translation: Add Text" {
          n651 = in-place {
            in-place-border: w1370 -> [w1374]
            n652 = in-place-cluster #14(w1372) -> ("T.Tr"=w1377:map{string, T14})
            n653 = in-place {
              n654 = in-place-map #15(w1377, w1374) -> ()  [unwired: 1 in, 2 out]
              n655 = in-place-map #15(T14 {"Tags"="", "Comment"="", "Properties"=[]} ("value"), LVMapReplaceAction."Add or Modify Entry" ("action")) -> (w1376:map{string, T14}, w1375:bool)  [unwired: 1 out]
            }
            n656 = case shown="True" w1375 {
              tunnel: w1374 -> [w1379 w1384]
              frame True {
                n657 = property on="ListOfTextTranslations" class="LstBox (strict)"() -> ("Item Names"=w1382:string[])  [unwired: 2 in, 2 out]
                n658 = Build Array (concatenate)(w1382, w1379) -> (w1380:string[])
                n659 = Array Size(array=w1380) -> (size(s)=w1378:i32)
                n660 = Decrement(x=w1378) -> (x-1=w1381:i32)
                n661 = property on="ListOfTextTranslations" class="LstBox (strict)"("Item Names"=w1380, "Val(Sgnl)"=w1381) -> ()  [unwired: 2 in, 2 out]
              }
              frame False {
                n662 = property on="ListOfTextTranslations" class="LstBox (strict)"() -> ("Item Names"=w1385:string[])  [unwired: 2 in, 2 out]
                n663 = Search 1D Array(1D array=w1385, element=w1384) -> (index of element=w1383:i32)  [unwired: 1 in]
                n664 = property on="ListOfTextTranslations" class="LstBox (strict)"("Val(Sgnl)"=w1383) -> ()  [unwired: 2 in, 2 out]
              }
            }
            n665 = in-place-cluster #14("T.Tr"=w1376) -> (w1371:T18)
          }
        }
        frame "Text Translation: Delete Text" {
          n666 = in-place {
            n667 = in-place-cluster #16(w1390) -> ("T.Tr"=w1396:map{string, T14})
            n668 = property on="ListOfTextTranslations" class="LstBox (strict)"() -> ("Item Names"=w1397:string[], "Value"=w1394:i32)  [unwired: 2 in, 2 out]
            n669 = Delete From Array(array=w1397, index=w1394) -> (deleted portion=w1392:string, array with subset deleted=w1393:string[])  [unwired: 1 in]
            n670 = Decrement(x=w1394) -> (x-1=w1398:i32)
            n671 = Remove From Map(10:w1392, 11:w1396) -> (3:w1395:map{string, T14})  [unwired: 2 out]
            n672 = property on="ListOfTextTranslations" class="LstBox (strict)"("Item Names"=w1393, "Val(Sgnl)"=w1398) -> ()  [unwired: 2 in, 2 out]
            n673 = in-place-cluster #16("T.Tr"=w1395) -> (w1389:T18)
          }
        }
        frame "Text Translation: Rename Text" {
          # "\"Old\" >> \"New\""
          n674 = in-place {
            in-place-border: w1400 -> [w1412]
            w1405 = TRUE ("replace all? (F)")
            w1404 = "\"" ("search string")
            n675 = in-place-cluster #17(w1402) -> ("T.Tr"=w1411:map{string, T14})
            n676 = call <vilib>:"Parse State Queue__JKI_lib_State_Machine.vi"("State Queue"=w1412) -> ("Current State"=w1406:string, "Arguments"=w1407:string)  [unwired: 12 in, 1 out]
            n677 = Search and Replace String(replace all?=w1405, input string=w1407, search string=w1404) -> (result string=w1408:string)  [unwired: 5 in, 3 out]
            n678 = Search and Replace String(replace all?=w1405, input string=w1406, search string=w1404) -> (result string=w1409:string)  [unwired: 5 in, 3 out]
            n679 = Look In Map(map=w1411, key=w1408) -> (key not found?=w1410:bool)  [unwired: 1 in, 1 out]
            n680 = case shown="False" w1410 {
              tunnel: [w1416 w1423] -> w1413
              tunnel: w1409 -> [w1414 w1419]
              tunnel: w1411 -> [w1416 w1418]
              tunnel: w1408 -> [_ w1417]
              frame False {
                # "Neuen Namen wieder entfernen!"
                n681 = local write "TextName"(w1414) -> ()
                n682 = One Button Dialog(message="Kann nicht umbenannt werden.\nEintrag existiert schon unter diesem Namen.") -> ()  [unwired: 1 in, 1 out]
              }
              frame True {
                n683 = Remove From Map(10:w1419, 11:w1418) -> (1:w1424:T14, 3:w1425:map{string, T14})  [unwired: 1 out]
                n684 = Insert Into Map(map in=w1425, key=w1417, value=w1424) -> (map out=w1423:map{string, T14})  [unwired: 2 out]
                n685 = for {
                  tunnel: w1423 -> [w1427] mode=indexing
                  tunnel: [w1426] -> w1421 mode=indexing
                  n686 = Unbundle By Name(w1427) -> ("Label"=w1426:string)
                }
                n687 = control-ref of="ListOfTextTranslations"() -> (w1422:refnum<vi>)
                n688 = Search 1D Array(1D array=w1421, element=w1417) -> (index of element=w1420:i32)  [unwired: 1 in]
                n689 = property on="Property Node" class="LstBox (strict)"(reference=w1422, "Item Names"=w1421, "Value"=w1420) -> ()  [unwired: 1 in, 2 out]
              }
            }
            n690 = in-place-cluster #17("T.Tr"=w1413) -> (w1401:T18)
          }
        }
        frame "Text Translation: Edit Properties" {
          n691 = Unbundle By Name(w1430) -> ("LT.Data.Languages"=w1429:cluster{"ANSI":string[], "Unicode":string[]})
          n692 = in-place {
            in-place-border: w1429 -> [w1438]
            w1436 = 0  # Language
            w1435 = "String Value_"  # Property
            w1440 = 1  # Text
            # "Is needed for compatibility with \ntree tag from Front Panel Translation.\nSee  \"FP Translation: Edit Properties\"."
            n693 = in-place-cluster #18(w1430) -> ("T.Tr"=w1444:map{string, T14})
            n694 = property on="TextTranslation" class="MCListbox (strict)"() -> ("ItemNames"=w1441:string[][], "Value"=w1437:i32)  [unwired: 2 in, 2 out]
            n695 = local read "TextName"() -> (w1442:string)
            n696 = Index Array(array=w1441, index (row) #1=w1437, index (col) #1=w1440, index (row) #2=w1437, index (col) #2=w1436) -> (element #1=w1439:string, element #2=w1434:string)
            n697 = Concatenate Strings(w1435, w1434) -> (w1433:string)
            n698 = call "Edit Property In Translation.vi"("Languages"=w1438, "Property_Language"=w1433, "Translations Text"=w1439, "Control Label Name"=w1442, "Translastions in"=w1444) -> ("Translastions out"=w1443:map{string, T14})  [unwired: 6 in]
            n699 = in-place-cluster #18("T.Tr"=w1443) -> (w1431:T18)
          }
        }
        frame "Text Translation: Filter" {
          n700 = Unbundle By Name(w1450) -> ("T.Tr"=w1449:map{string, T14})
          n701 = for {
            tunnel: w1449 -> [w1455] mode=indexing
            tunnel: [w1454] -> w1448 mode=indexing
            n702 = Unbundle By Name(w1455) -> ("Label"=w1454:string)
          }
          n703 = To Lower Case(string="Search text") -> (all lower case string=w1451:string)
          n704 = Empty String/Path?(string/path=w1451) -> (empty?=w1452:bool)
          n705 = for {
            tunnel: w1448 -> [w1456] mode=indexing
            tunnel: [w1464] -> w1445 mode=indexing if=w1462
            tunnel: w1451 -> [w1463]
            tunnel: w1452 -> [w1458]
            n706 = To Lower Case(string=w1456) -> (all lower case string=w1457:string)
            n707 = Match Pattern(string=w1457, regular expression=w1463) -> (offset past match=w1461:i32)  [unwired: 1 in, 3 out]
            n708 = Greater Or Equal To 0?(x=w1461) -> (x >= 0?=w1460:bool)
            n709 = Or(x=w1460, y=w1458) -> (x .or. y?=w1459:bool)
            n710 = case shown="True" w1459 {
              tunnel: [_ w1465] -> w1464
              tunnel: [_ TRUE] -> w1462
              tunnel: w1456 -> [_ w1465]
              frame False {
              }
              frame True {
              }
            }
          }
          n711 = property on="ListOfTextTranslations" class="LstBox (strict)"("Item Names"=w1445) -> ()  [unwired: 2 in, 2 out]
        }
      }
      n712 = call <vilib>:"Add State(s) to Queue__JKI_lib_State_Machine.vi"("State(s) in Front (\"\")"=w368, "State(s) in (\"\")"=w371, "State(s) at Back (\"\")"=w369) -> ("States Out"=w370:string)  [unwired: 12 in]
    }
  }
  "error out" <- "error in (no error)"
